vi "HOST.vi"() -> ()   [LabVIEW 2018]
uses:
  <vilib>/userdefined/High Color/nirio_resource_hc.ctl
  <instrlib>/niDCPower/nidcpower.llb/niDCPower Measurement Type.ctl
  <vilib>/FPGAPlugInAG/PXI-7953R/niLvFpga_Open_PXI-7953R.vi
  <vilib>/rvi/interface/common/dynamic/niFpgaDynamicAddResources.vi
  <vilib>/FPGAPlugInAG/Dynamic/niLvFpga_Reset_Dynamic.vi
  <vilib>/FPGAPlugInAG/Dynamic/niLvFpga_Run_Dynamic.vi
  <vilib>/Utility/error.llb/Error Cluster From Error Code.vi
  <vilib>/rvi/errors/niLvFpgaAdjustHostInterfaceError.vi
  <vilib>/FPGAPlugInAG/Dynamic/niLvFpga_Close_Dynamic.vi
  <vilib>/rvi/interface/nirviOpenFPGA/nirviOpenFPGA.xnode
  FPGA Bitfiles/KAI02050_FPGATarget_TARGET_lLVpfqL41SY.lvbitx
  <vilib>/rvi/interface/nirviMethod/nirviMethod.xnode
  <vilib>/rvi/interface/nirviReadWriteControl/nirviReadWriteControl.xnode
  <vilib>/rvi/interface/nirviCloseFPGA/nirviCloseFPGA.xnode
  NiFpgaLv.dll
  <vilib>/rvi/interface/Simulation/niFpgaSimulationCallBeginRW.vi
  <vilib>/FPGAPlugInAG/Dynamic/niLvFpga_ReadFifo_Dynamic.vi
  <vilib>/rvi/errors/niLvFpgaMergeErrorWithErrorCode.vi
panel:
  in  "LED":bool caption="output enabled"
  out "Eh":dbl
  out "Ev":dbl
  out "D, дБ":dbl
  in  "Uнас, мВ":dbl
  in  "Расчет":bool
  out "Nбд":u32
  out "Nчд":u32
  out "Картинка":bool
  out "PRNU, %":dbl
  out "DSNU, мВ, p-p":dbl
  in  "Частота, МГц?":u16=40
  in  "ISO":u16=1
  out "Vout, мВ":dbl
  in  "FPGA":T1="PXI1Slot6"
  out "Тнак, мс":dbl
  in  "Светлый (T)\nТемный (F)":bool
  in  "Frames":path=path "C:/VPL/LabView_PRJ/KAI02050/FRAMES"
  in  "ПРИМЕЧАНИЕ":string
  in  "SAVE":bool
  out "Элем.":u32
  out "Записали FIFO":bool
  out "R_LOW_char":dbl(graph)=0.00522832579698275
  out "VSUB_char":dbl(graph)=-7.684341850864879e-08
  out "STAB-15_char":dbl(graph)=0.00521525227136925
  out "STAB+15_char":dbl(graph)=-1.545303562529033e-05
  out "LED_char":dbl(graph)=5.756096264886238e-05
  out "OG_char":dbl(graph)=7.305007030606659e-07
  out "VDD_char":dbl(graph)=-4.908628444273266e-07
  out "ESD_char":dbl(graph)=-2.550812858562396e-06
  out "RD_char":dbl(graph)=-3.2917542324318195e-07
  out "ADC_char":dbl(graph)=-0.007202656860577676
  in  "MOVIE":bool
  out "Image":T2(plugin-control)
  in  "For FIFO (79)":i32=79
  out "Data":u8[][](array[numeric])
  in  "54592":u32=54592
  in  "FRAME!":bool
  in  "17850?":u16=17850
  in  "SUB2":u16=750
  in  "SUB1":u16=550
  in  "Номер SUB":u16=3
  in  "P4B_2@":u16=1700
  in  "P4B_1@":u16=1100
  in  "P4B_2@@":u16=2600
  in  "P4B_1@@":u16=2000
  in  "P1B_2_2":u16=2000
  in  "P1B_2_1":u16=1700
  in  "P1B_1_2":u16=250
  in  "P1B_1_1":u16=50
  in  "P1B_1_2@":u16=2500
  in  "P1B_1_1@":u16=1000
  in  "P4B_2":u16=350
  in  "P4B_1":u16=150
  in  "P3B_2":u16=245
  in  "P3B_1":u16=55
  in  "P3B_2@":u16=2500
  in  "P3B_1@":u16=1000
  in  "P2B_2@":u16=2600
  in  "P2B_1@":u16=1100
  in  "P2B_1":u16=155
  in  "P2B_2":u16=345
  in  "0":u16
  in  "CDS1_1":u8=1
  in  "CDS1_2":u8=4
  in  "CDS2_1":u8=5
  in  "CDS2_2":u8=10
  in  "ADC_1":u8=1
  in  "ADC_2":u8=6
  in  "17846?":u16=17846
  in  "789?":u16=789
  in  "17860?":u16=17860
  in  "P5_1":u8
  in  "P5_2":u8=6
  in  "P6_1":u8
  in  "P6_2":u8=6
  in  "P7_1":u8
  in  "P7_2":u8=2
  in  "P_end":u8=10
  in  "С_1265?":u16=1265
  in  "HIGH":u8=6
  in  "LOW":u8=1
  in  "Между кадрами, мс":u16
  in  "А(T)/А+В(F)":bool=TRUE
  in  "Линейки":bool
  in  "1":u8
  in  "2":u8
  out "Данные":u8
  in  "Направление бит":bool
  in  "4":refnum<k15>="PXI1Slot5_2" caption="1"
  in  "3":refnum<k15>="PXI1Slot4" caption="1"
  in  "2":refnum<k15>="PXI1Slot3" caption="1"
  in  "1":refnum<k15>="PXI1Slot2"
  in  "SIM_SEL":bool
  in  "R_LOW_selcur":dbl=0.01 caption="current limit" format="%_6p"
  in  "VSUB_selcur":dbl=0.01 caption="current limit" format="%_6p"
  in  "STAB-15_selcur":dbl=0.07 caption="current limit" format="%_6p"
  in  "STAB+15_selcur":dbl=0.10000000000000003 caption="current limit" format="%_6p"
  in  "LED_selcur":dbl=0.09 caption="current limit" format="%_6p"
  in  "OG_selcur":dbl=0.01 caption="current limit" format="%_6p"
  in  "VDD_selcur":dbl=0.04 caption="current limit" format="%_6p"
  in  "ESD_selcur":dbl=0.01 caption="current limit" format="%_6p"
  in  "RD_selcur":dbl=0.009999999999999997 caption="current limit" format="%_6p"
  in  "ADC_selcur":dbl=0.17 caption="current limit" format="%_6p"
  out "R_LOW":u16
  out "VSUB":u16
  out "STAB-15":u16
  out "STAB+15":u16
  out "LED":u16
  out "OG":u16
  out "VDD":u16
  out "ESD":u16
  out "RD":u16
  out "ADC":u16
  out "R_LOW":bool
  out "VSUB":bool
  out "STAB-15":bool
  out "STAB+15":bool
  out "LED":bool
  out "OG":bool
  out "VDD":bool
  out "ESD":bool
  out "RD":bool
  out "ADC":bool
  in  "Прошить АЦП":bool
  out "АЦП прошит!":bool
  in  "Какой канал?":enum16{"GREEN", "RED", "BLUE"}(ring)=enum."BLUE"
  in  "Усиление (до 6)_RED":u8=1
  in  "Усиление (до 6)_BLUE":u8=1
  in  "Усиление (до 6)_GREEN":u8=1
  in  "Смещение, до 300_BLUE":dbl
  in  "+/- BLUE":enum16{"-", "+"}(ring)=enum."+"
  in  "Смещение, до 300_RED":dbl
  in  "+/- RED":enum16{"-", "+"}(ring)=enum."+"
  in  "Смещение, до 300_GREEN":dbl
  in  "+/- GREEN":enum16{"-", "+"}(ring)=enum."+"
  in  "2/4 V":enum16{"2V", "4V"}(ring)
  in  "3CH/1CH":enum16{"3CH", "1CH"}(ring)=enum."1CH"
  out "Configuration":bool[](array[boolean])
  out "R_LOW_cur":dbl caption="measurement" format="%_6g"
  in  "R_LOW_curlim":dbl=0.015 caption="current limit" format="%_6p"
  in  "R_LOW, V":dbl=-2.0 caption="voltage level" format="%_6p"
  out "VSUB_cur":dbl caption="measurement" format="%_6g"
  in  "VSUB_curlim":dbl=0.015 caption="current limit" format="%_6p"
  in  "VSUB, V":dbl=8.0 caption="voltage level" format="%_6p"
  in  "ADC, V":dbl=6.0 caption="voltage level" format="%_6p"
  in  "VDD, V":dbl=14.900000000000004 caption="voltage level" format="%_6p"
  in  "OG, V":dbl=-2.0 caption="voltage level" format="%_6p"
  in  "STAB+15, V":dbl=15.0 caption="voltage level" format="%_6p"
  in  "ADC_curlim":dbl=0.2 caption="current limit" format="%_6p"
  in  "RD_curlim":dbl=0.045000000000000005 caption="current limit" format="%_6p"
  in  "VDD_curlim":dbl=0.1 caption="current limit" format="%_6p"
  in  "OG_curlim":dbl=0.015 caption="current limit" format="%_6p"
  in  "LED_curlim":dbl=0.1 caption="current limit" format="%_6p"
  in  "STAB+15_curlim":dbl=0.6 caption="current limit" format="%_6p"
  out "ADC_cur":dbl caption="measurement" format="%_6g"
  out "RD_cur":dbl caption="measurement" format="%_6g"
  out "VDD_cur":dbl caption="measurement" format="%_6g"
  out "OG_cur":dbl caption="measurement" format="%_6g"
  out "LED_cur":dbl caption="measurement" format="%_6g"
  out "STAB+15_cur":dbl caption="measurement" format="%_6g"
  in  "RD, V":dbl=12.0 caption="voltage level" format="%_6p"
  in  "LED, V":dbl caption="voltage level" format="%_6p"
  in  "ESD_curlim":dbl=0.015 caption="current limit" format="%_6p"
  out "ESD_cur":dbl caption="measurement" format="%_6g"
  in  "ESD, V":dbl=-9.0 caption="voltage level" format="%_6p"
  in  "STAB-15, V":dbl=-15.0 caption="voltage level" format="%_6p"
  in  "STAB-15_curlim":dbl=0.1 caption="current limit" format="%_6p"
  out "STAB-15_cur":dbl caption="measurement" format="%_6g"
  in  "Питание":bool
  in  "Стоп":bool
  out "Температура":string="0"
  in  "LOGS":path=path "C:/VPL/LabView_PRJ/KAI02050/LOGS"
  out "Номер образца":string="0"
  out "Analis":u16[][](array[numeric])
  # "ДЛЯ ТЗЧ ОПТИМАЛКА - 6 5 10 6"
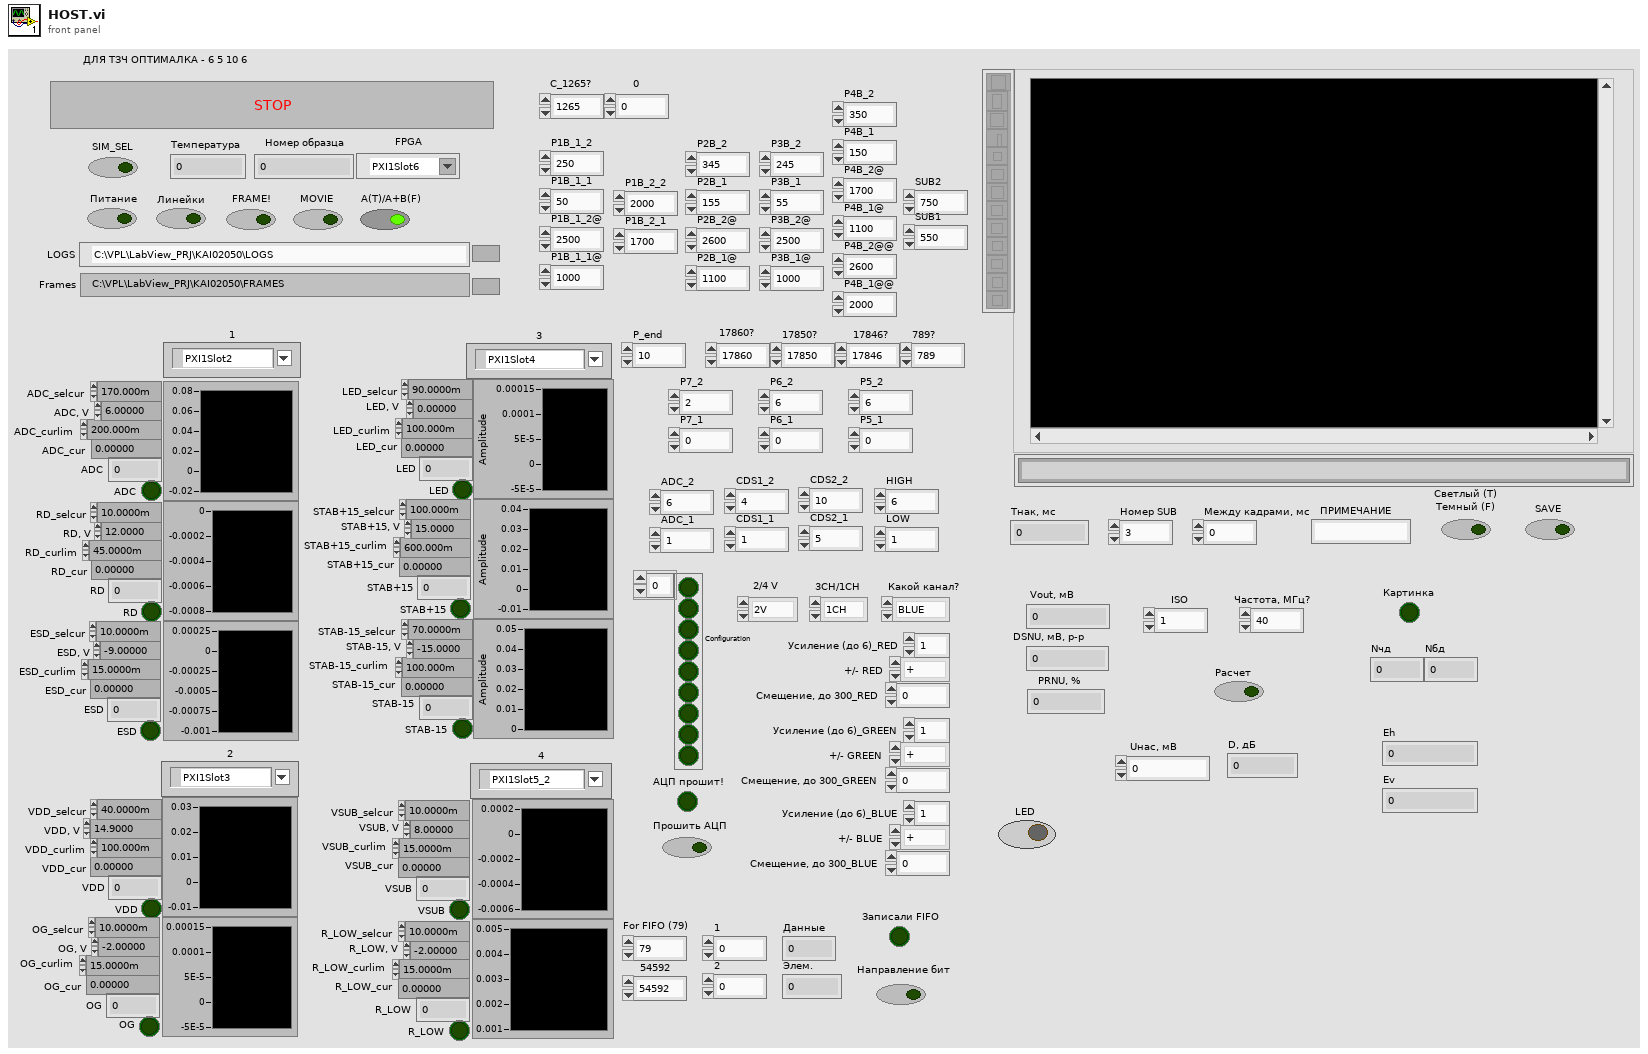
[diagram p1: front panel]
types:
  T1 = typedef "nirio_resource_hc.ctl" = tag
  T2 = typedef "IMAQ Image.ctl" = refnum<image>
  T3 = typedef "Image Type" = u32
  T4 = enum16{"open", "replace", "create", "open or create", "replace or create", "replace or create with confirmation"}
  T5 = enum16{"Configuration", "MUX", "RED PGA", "GREEN PGA", "BLUE PGA", "RED OFF", "GREEN OFF", "BLUE OFF"}
  T6 = typedef "niDCPower Measurement Type.ctl" = i32
  T7 = cluster{"Global Rectangle":i32[], "Contours":cluster{"Contour Type":u32, "ROI Type":u32, "Points":i32[]}[]}
  T8 = cluster{"Contour Type":u32, "ROI Type":u32, "Points":i32[]}[]
  T9 = cluster{"Contour Type":u32, "ROI Type":u32, "Points":i32[]}
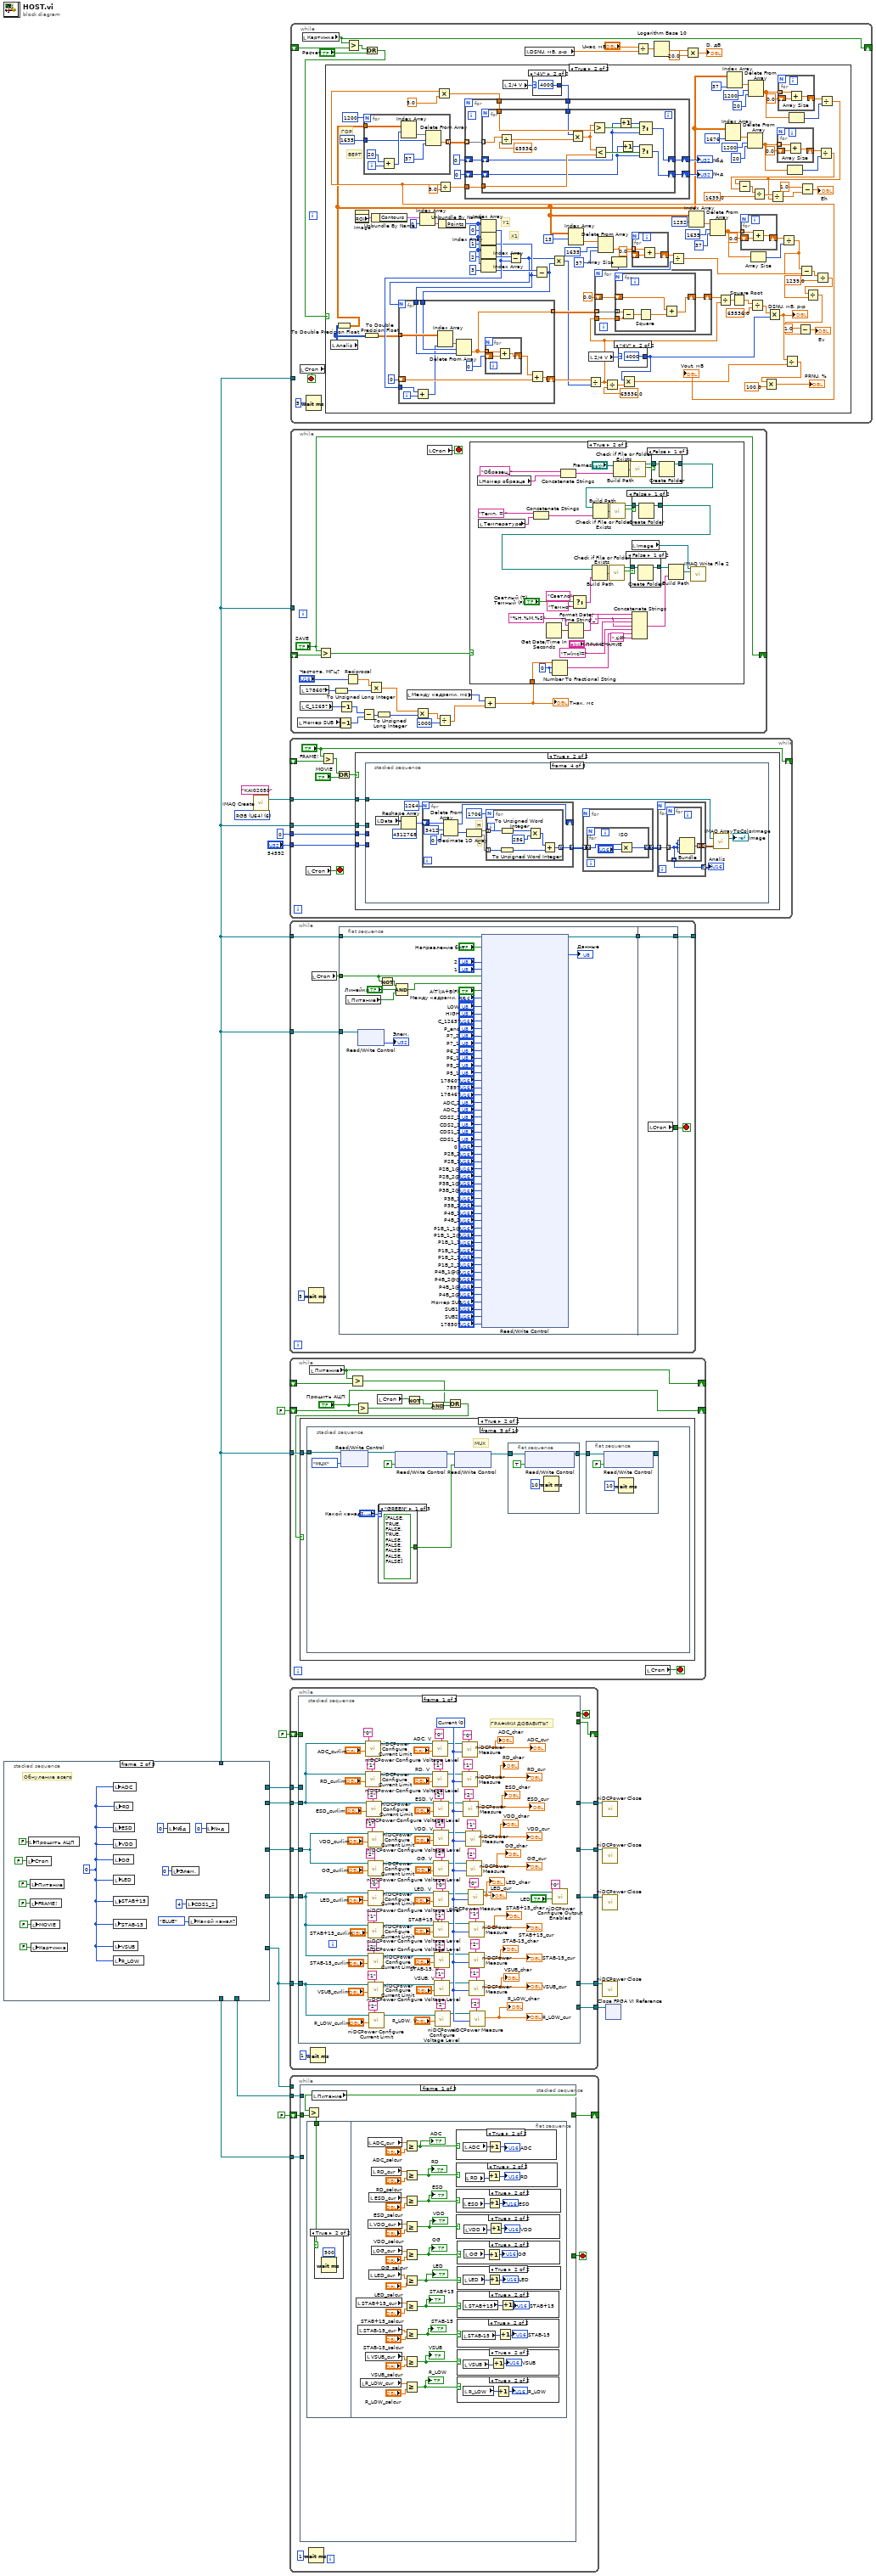
[diagram p0: block diagram]
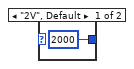
[diagram p3: hidden frame]
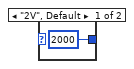
[diagram p4: hidden frame]
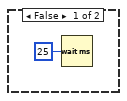
[diagram p5: hidden frame]
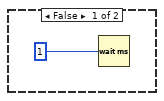
[diagram p9: hidden frame]
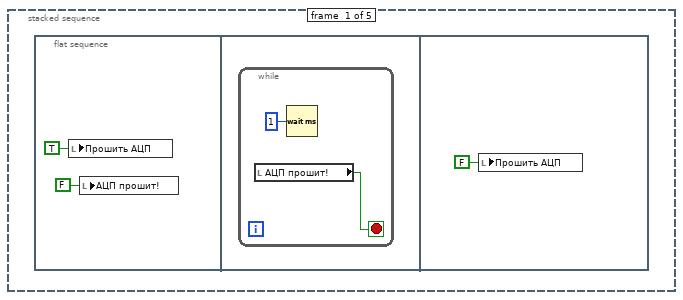
[diagram p10: hidden frame]
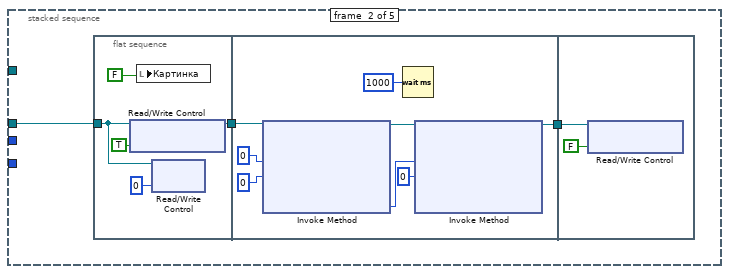
[diagram p11: hidden frame]
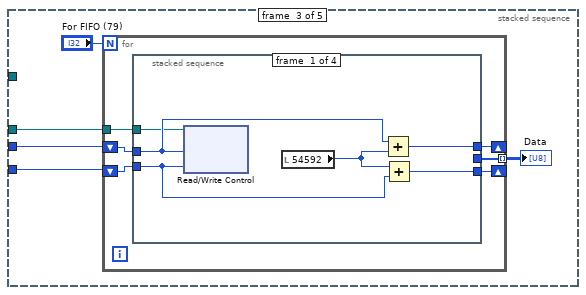
[diagram p12: hidden frame]
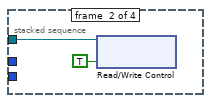
[diagram p13: hidden frame]
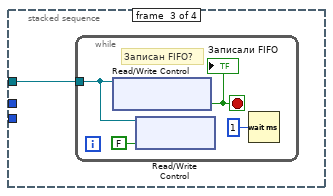
[diagram p14: hidden frame]
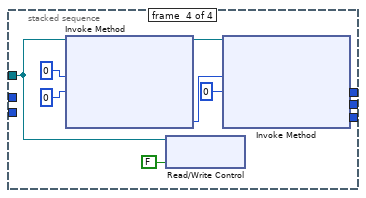
[diagram p15: hidden frame]
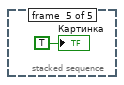
[diagram p16: hidden frame]
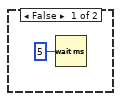
[diagram p17: hidden frame]
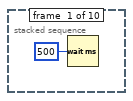
[diagram p18: hidden frame]
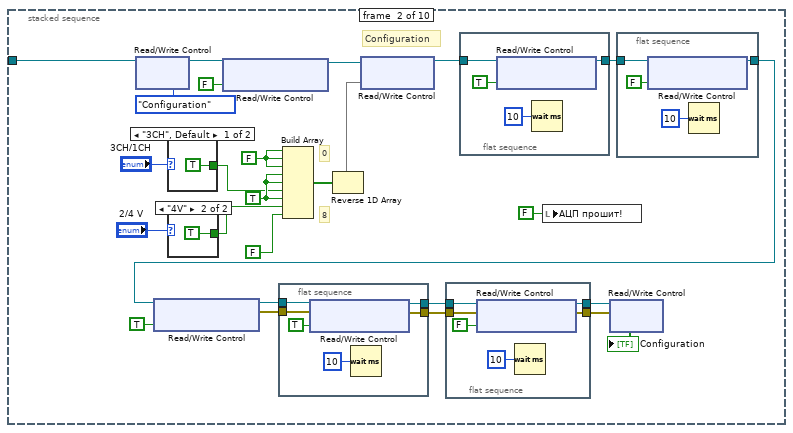
[diagram p19: hidden frame]
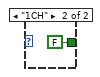
[diagram p20: hidden frame]
diagram:
  w3 = T3 6 items=["Grayscale (U8)", "Grayscale (I16)", "Grayscale (SGL)", "Complex (CSG)", "RGB (U32)", "HSL (U32)", "RGB (U64)"] ("Image Type")
  n1 = stacked-sequence {
    tunnel: [_ _ _ w83 _] -> w18
    tunnel: [_ _ _ _ w99] -> w19
    tunnel: [_ _ _ _ w98] -> w21
    tunnel: [_ _ _ _ w97] -> w20
    tunnel: [_ _ _ w83 _] -> w4
    tunnel: [_ _ _ w83 _] -> w9
    tunnel: [_ _ w49 _ _] -> w10
    tunnel: [_ _ _ _ w93] -> w11
    frame #0 {
      n2 = call "Begin.vi"() -> ("Температура 2"=→"Температура":string, "Номер образца 2"=→"Номер образца":string)  [unwired: 10 in]
    }
    frame #1 {
      w32 = u16 0 ("ADC")
      # "Обнуление всего"
      n3 = local write "Стоп"(FALSE ("Стоп")) -> ()
      n4 = local write "Прошить АЦП"(FALSE ("Прошить АЦП")) -> ()
      n5 = local write "Питание"(FALSE ("Питание")) -> ()
      n6 = local write "FRAME!"(FALSE ("FRAME!")) -> ()
      n7 = local write "MOVIE"(FALSE ("MOVIE")) -> ()
      n8 = local write "Картинка"(FALSE ("Картинка")) -> ()
      n9 = local write "ADC"(w32) -> ()
      n10 = local write "STAB-15"(w32) -> ()
      n11 = local write "VSUB"(w32) -> ()
      n12 = local write "ESD"(w32) -> ()
      n13 = local write "VDD"(w32) -> ()
      n14 = local write "OG"(w32) -> ()
      n15 = local write "LED"(w32) -> ()
      n16 = local write "STAB+15"(w32) -> ()
      n17 = local write "R_LOW"(w32) -> ()
      n18 = local write "RD"(w32) -> ()
      n19 = local write "Nбд"(0 ("Nбд")) -> ()
      n20 = local write "Элем."(u32 0 ("Элем.")) -> ()
      n21 = local write "CDS1_2"(u8 4 ("CDS1_2")) -> ()
      n22 = local write "Какой канал?"(enum16{"GREEN", "RED", "BLUE"}."BLUE" ("Какой канал?")) -> ()
      n23 = local write "Nчд"(0 ("Nчд")) -> ()
    }
    frame #2 {
      w37 = "\t"
      n24 = local read "Номер образца"() -> (w71:string)
      n25 = Build Path(base path="LOGS", name or relative path=w71) -> (appended path=w68:path)
      n26 = Get Date/Time In Seconds() -> (seconds since 1Jan1904=w65:timestamp)
      n27 = call <vilib>:"Check if File or Folder Exists.vi"("path"=w68) -> ("file or folder exists?"=w69:bool, "dup path"=w70:path)  [unwired: 8 in, 1 out]
      n28 = local read "Температура"() -> (w44:string)
      n29 = Format Date/Time String(time format string (%c)="%d %H.%M.%S", seconds (now)=w65) -> (date/time string=w63:string)  [unwired: 1 in]
      n30 = case shown="False" w69 {
        tunnel: w70 -> [w80 w81]
        tunnel: [w79 w81] -> w45
        frame False {
          n31 = Create Folder(path (use dialog)=w80) -> (created path=w79:path)  [unwired: 2 in, 2 out]
        }
        frame True {
        }
      }
      n32 = Concatenate Strings(w63, ".xls" ("string")) -> (w62:string)
      n33 = Build Path(base path=w45, name or relative path=w44) -> (appended path=w48:path)
      n34 = call <vilib>:"Check if File or Folder Exists.vi"("path"=w48) -> ("file or folder exists?"=w47:bool, "dup path"=w46:path)  [unwired: 8 in, 1 out]
      n35 = case shown="False" w47 {
        tunnel: w46 -> [w73 w74]
        tunnel: [w72 w74] -> w43
        frame False {
          n36 = Create Folder(path (use dialog)=w73) -> (created path=w72:path)  [unwired: 2 in, 2 out]
        }
        frame True {
        }
      }
      n37 = Build Path(base path=w43, name or relative path=w62) -> (appended path=w64:path)
      n38 = Open/Create/Replace File(file path (use dialog)=w64, operation (0:open)=T4."open or create", access (0:read/write)=enum16{"read/write", "read-only", "write-only"}."read/write") -> (refnum out=w66:refnum<file>)  [unwired: 3 in, 2 out]
      n39 = case shown="True" TRUE {
        tunnel: w66 -> [w75 w78]
        tunnel: [w75 w76] -> w61
        frame False {
        }
        frame True {
          n40 = Set File Position(refnum=w78, from (0:start)=enum16{"start", "end", "current"}."end") -> (refnum out=w76:refnum<file>)  [unwired: 2 in, 1 out]
        }
      }
      n41 = Format Into String(initial string=w61, "Time" ("input 1"), w37, "ADC_cur", w37, "RD_cur", w37, "ESD_cur", w37, "VDD_cur", w37, "OG_cur", w37, "LED_cur", w37, "STAB+15_cur", w37, "STAB-15_cur", w37, "VSUB_cur", w37, "R_LOW_cur", w37, "\r\n") -> (resulting string=w49:refnum<file>)  [unwired: 2 in, 1 out]
    }
    frame #3 {
      n42 = xnode "Open FPGA VI Reference"("resource name"="FPGA") -> ("FPGA VI Reference Out"=w84:refnum<k20>, "error out"=w86:errorcluster)  [unwired: 1 in]
      n43 = xnode "Invoke Method"("FPGA VI Reference In"=w84, "error in"=w86) -> ("FPGA VI Reference Out"=w87:refnum<k20>, "error out"=w85:errorcluster)
      n44 = xnode "Invoke Method"("FPGA VI Reference In"=w87, "error in"=w85) -> ("FPGA VI Reference Out"=w83:refnum<k20>)  [unwired: 1 in, 1 out]
    }
    frame #4 {
      n45 = call <instrlib>:"niDCPower Initialize.vi"("resource name"="3") -> ("error out"=w105:errorcluster, "instrument handle out"=w102:refnum<k15>)  [unwired: 3 in, 6 out]
      n46 = call <instrlib>:"niDCPower Initialize.vi"("resource name"="2") -> ("error out"=w103:errorcluster, "instrument handle out"=w100:refnum<k15>)  [unwired: 3 in, 6 out]
      n47 = call <instrlib>:"niDCPower Initialize.vi"("resource name"="4") -> ("error out"=w95:errorcluster, "instrument handle out"=w96:refnum<k15>)  [unwired: 3 in, 6 out]
      n48 = call <instrlib>:"niDCPower Initialize.vi"("resource name"="1") -> ("error out"=w104:errorcluster, "instrument handle out"=w101:refnum<k15>)  [unwired: 3 in, 6 out]
      n49 = call <instrlib>:"niDCPower Configure Voltage Level.vi"("error in (no error)"=w105, "voltage level"=0.0, "channel name"="0,1,2", "instrument handle"=w102) -> ("instrument handle out"=w99:refnum<k15>)  [unwired: 6 in, 1 out]
      n50 = call <instrlib>:"niDCPower Configure Voltage Level.vi"("error in (no error)"=w103, "voltage level"=0.0, "channel name"="0,1,2", "instrument handle"=w100) -> ("instrument handle out"=w97:refnum<k15>)  [unwired: 6 in, 1 out]
      n51 = call <instrlib>:"niDCPower Configure Voltage Level.vi"("error in (no error)"=w95, "voltage level"=0.0, "channel name"="0,1,2", "instrument handle"=w96) -> ("instrument handle out"=w93:refnum<k15>)  [unwired: 6 in, 1 out]
      n52 = call <instrlib>:"niDCPower Configure Voltage Level.vi"("error in (no error)"=w104, "voltage level"=0.0, "channel name"="0,1,2", "instrument handle"=w101) -> ("instrument handle out"=w98:refnum<k15>)  [unwired: 6 in, 1 out]
    }
  }
  n53 = call "IMAQ Create"("Image Name"="KAI02050", "Image Type"=w3) -> ("New Image"=w1:T2)  [unwired: 3 in, 1 out]
  n54 = while {
    tunnel: w4 -> [w118]
    shift-right: ["FRAME!"] -> _
    shift-left: _ -> [w120]
    tunnel: u32 0 -> [w117]
    tunnel: "54592" -> [w116]
    tunnel: w1 -> [w112]
    stop <- w121 stop-if-true
    n55 = local read "Стоп"() -> (w121:bool)
    n56 = Greater?(x="FRAME!", y=w120) -> (0:w114:bool)
    n57 = Or(x=w114, y="MOVIE") -> (x .or. y?=w115:bool)
    n58 = case shown="True" w115 {
      tunnel: w118 -> [_ w126]
      tunnel: w117 -> [_ w125]
      tunnel: w116 -> [_ w124]
      tunnel: w112 -> [_ w123]
      frame False {
        n59 = Wait (ms)(milliseconds to wait=u32 1) -> ()  [unwired: 1 out]
      }
      frame True {
        n60 = stacked-sequence {
          tunnel: w126 -> [_ w134 w154 _ _]
          tunnel: w125 -> [_ _ w153 _ _]
          tunnel: w124 -> [_ _ w152 _ _]
          tunnel: w123 -> [_ _ _ w191 _]
          frame #0 {
            n61 = flat-sequence {
              frame #0 {
                n62 = local write "Прошить АЦП"(TRUE ("Прошить АЦП")) -> ()
                n63 = local write "АЦП прошит!"(FALSE ("АЦП прошит!")) -> ()
              }
              frame #1 {
                n64 = while {
                  stop <- w130 stop-if-true
                  n65 = local read "АЦП прошит!"() -> (w130:bool)
                  n66 = Wait (ms)(milliseconds to wait=u32 1) -> ()  [unwired: 1 out]
                }
              }
              frame #2 {
                n67 = local write "Прошить АЦП"(FALSE ("Прошить АЦП")) -> ()
              }
            }
          }
          frame #1 {
            n68 = flat-sequence {
              tunnel: w134 -> [w138]
              tunnel: [w139] -> w133
              tunnel: w133 -> [w141]
              tunnel: [w140] -> w132
              tunnel: w132 -> [w148]
              frame #0 {
                n69 = xnode "Read/Write Control"("FPGA VI Reference In"=w138, "Кадр в память"=TRUE) -> ("FPGA VI Reference Out"=w139:refnum<k20>)  [unwired: 1 in, 1 out]
                n70 = local write "Картинка"(FALSE ("Картинка")) -> ()
                n71 = xnode "Read/Write Control"("FPGA VI Reference In"=w138, "Элем."=u32 0) -> ()  [unwired: 1 in, 2 out]
              }
              frame #1 {
                n72 = xnode "Invoke Method"("FPGA VI Reference In"=w141, "Number of Elements"=u32 0, "Timeout (ms)"=0) -> ("FPGA VI Reference Out"=w146:refnum<k20>, "Elements Remaining"=w145:u32)  [unwired: 1 in, 2 out]
                n73 = Wait (ms)(milliseconds to wait=u32 1000) -> ()  [unwired: 1 out]
                n74 = xnode "Invoke Method"("FPGA VI Reference In"=w146, "Number of Elements"=w145, "Timeout (ms)"=0) -> ("FPGA VI Reference Out"=w140:refnum<k20>)  [unwired: 1 in, 3 out]
              }
              frame #2 {
                n75 = xnode "Read/Write Control"("FPGA VI Reference In"=w148, "Кадр в память"=FALSE) -> ()  [unwired: 1 in, 2 out]
              }
            }
          }
          frame #2 {
            n76 = for {
              N: "For FIFO (79)" -> [_]
              shift-right: [w158] -> _
              shift-left: w153 -> [w160]
              shift-right: [w157] -> _
              shift-left: w152 -> [w159]
              tunnel: w154 -> [w156]
              tunnel: [w155] -> w151 mode=indexing
              n77 = stacked-sequence {
                tunnel: [_ _ _ w179] -> w155
                tunnel: [w166 _ _ _] -> w158
                tunnel: [w165 _ _ _] -> w157
                tunnel: w160 -> [w163 _ _ _]
                tunnel: w159 -> [w164 _ _ _]
                tunnel: w156 -> [w162 w167 w169 w174]
                frame #0 {
                  n78 = xnode "Read/Write Control"("FPGA VI Reference In"=w162, "Нач_адр"=w163, "Кон_адр"=w164) -> ()  [unwired: 1 in, 2 out]
                  n79 = local read "54592"() -> (w161:u32)
                  n80 = Add(x=w163, y=w161) -> (x+y=w166:u32)
                  n81 = Add(x=w161, y=w164) -> (x+y=w165:u32)
                }
                frame #1 {
                  n82 = xnode "Read/Write Control"("FPGA VI Reference In"=w167, "Кадр на ПК"=TRUE ("HOST")) -> ()  [unwired: 1 in, 2 out]
                }
                frame #2 {
                  n83 = while {
                    tunnel: w169 -> [w170]
                    stop <- w173 stop-if-true
                    # "Записан FIFO?"
                    n84 = xnode "Read/Write Control"("FPGA VI Reference In"=w170) -> ("Записали FIFO"=w173:bool)  [unwired: 1 in, 2 out]
                    "Записали FIFO" <- w173
                    n85 = xnode "Read/Write Control"("FPGA VI Reference In"=w170, "Кадр на ПК"=FALSE ("HOST")) -> ()  [unwired: 1 in, 2 out]
                    n86 = Wait (ms)(milliseconds to wait=u32 1) -> ()  [unwired: 1 out]
                  }
                }
                frame #3 {
                  n87 = xnode "Invoke Method"("FPGA VI Reference In"=w174, "Number of Elements"=u32 0, "Timeout (ms)"=0) -> ("FPGA VI Reference Out"=w180:refnum<k20>, "Elements Remaining"=w181:u32)  [unwired: 1 in, 2 out]
                  n88 = xnode "Read/Write Control"("FPGA VI Reference In"=w174, "Кадр на ПК"=FALSE ("HOST")) -> ()  [unwired: 1 in, 2 out]
                  n89 = xnode "Invoke Method"("FPGA VI Reference In"=w180, "Number of Elements"=w181, "Timeout (ms)"=0) -> ("Data"=w179:u8[])  [unwired: 1 in, 3 out]
                }
              }
            }
            "Data" <- w151
          }
          frame #3 {
            n90 = local read "Data"() -> (w190:u8[][])
            n91 = Reshape Array(w190, 4312768 ("dimension size")) -> (w187:u8[])
            n92 = for {
              N: 1264 -> [_]
              shift-right: [w206] -> _
              shift-left: w187 -> [w210]
              tunnel: [w202] -> w184 mode=indexing
              # "L"
              # "H"
              n93 = Delete From Array(array=w210, length=3412, index=0) -> (deleted portion=w207:u8[], array with subset deleted=w206:u8[])
              n94 = Decimate 1D Array(w207) -> (w205:u8[], w204:u8[])
              n95 = for {
                N: 1706 -> [_]
                tunnel: w205 -> [w216] mode=indexing
                tunnel: w204 -> [w217] mode=indexing
                tunnel: [w215] -> w202 mode=indexing
                n96 = To Unsigned Word Integer(number=w217) -> (unsigned 16bit integer=w211:u16)
                n97 = To Unsigned Word Integer(number=w216) -> (unsigned 16bit integer=w213:u16)
                n98 = Multiply(x=w213, y=u16 256) -> (x*y=w212:u16)
                n99 = Add(x=w212, y=w211) -> (x+y=w215:u16)
              }
            }
            n100 = for {
              tunnel: w184 -> [w193] mode=indexing
              tunnel: [w192] -> w183 mode=indexing
              n101 = for {
                tunnel: w193 -> [w196] mode=indexing
                tunnel: [w195] -> w192 mode=indexing
                n102 = Multiply(x="ISO", y=w196) -> (x*y=w195:u16)
              }
            }
            n103 = for {
              tunnel: [w199] -> w188 mode=indexing
              tunnel: w183 -> [w198] mode=indexing
              tunnel: [w197] -> w185 mode=indexing
              n104 = for {
                tunnel: w198 -> [w200] mode=indexing
                tunnel: [w201] -> w199 mode=indexing
                tunnel: [w200] -> w197 mode=indexing
                n105 = Bundle(w200, w200, w200, w200) -> (w201:cluster{u16, u16, u16, u16})  [unwired: 1 in]
              }
            }
            "Analis" <- w185
            n106 = call "IMAQ ArrayToColorImage"("Image"=w191, "Image Pixels (U64)"=w188) -> ("Image Out"=→"Image":T2)  [unwired: 3 in, 1 out]
          }
          frame #4 {
            "Картинка" <- TRUE
          }
        }
      }
    }
  }
  n107 = while {
    tunnel: w4 -> [w224]
    tunnel: [w223] -> _
    tunnel: w4 -> [w219]
    stop <- w220 stop-if-true
    n108 = Wait (ms)(milliseconds to wait=u32 5) -> ()  [unwired: 1 out]
    n109 = local read "Стоп"() -> (w222:bool)
    n110 = flat-sequence {
      tunnel: w224 -> [w282]
      tunnel: w222 -> [w229]
      tunnel: [w233] -> w221
      tunnel: w219 -> [w227]
      tunnel: [w286] -> w223
      tunnel: w221 -> [w286]
      tunnel: [w285] -> w220
      frame #0 {
        n111 = local read "Питание"() -> (w231:bool)
        n112 = xnode "Read/Write Control"("FPGA VI Reference In"=w227) -> ("Элем."=→"Элем.":u32)  [unwired: 1 in, 2 out]
        n113 = Not(x=w229) -> (.not. x?=w230:bool)
        n114 = Compound Arithmetic op=AND(w230, "Линейки", w231) -> (w228:bool)
        n115 = xnode "Read/Write Control"("FPGA VI Reference In"=w282, "Направление бит"="Направление бит", "2"="2", "1"="1", "Остановка основного цикла"=w229, "Линейки"=w228, "А(T)/А+В(F)"="А(T)/А+В(F)", "Между кадрами"="Между кадрами, мс", "LOW"="LOW", "HIGH"="HIGH", "С_1265?"="С_1265?", "P_end"="P_end", "P7_2"="P7_2", "P7_1"="P7_1", "P6_2"="P6_2", "P6_1"="P6_1", "P5_2"="P5_2", "P5_1"="P5_1", "17860?"="17860?", "789?"="789?", "17846?"="17846?", "ADC_2"="ADC_2", "ADC_1"="ADC_1", "CDS2_2"="CDS2_2", "CDS2_1"="CDS2_1", "CDS1_2"="CDS1_2", "CDS1_1"="CDS1_1", "0"="0", "P2B_2"="P2B_2", "P2B_1"="P2B_1", "P2B_1@"="P2B_1@", "P2B_2@"="P2B_2@", "P3B_1@"="P3B_1@", "P3B_2@"="P3B_2@", "P3B_1"="P3B_1", "P3B_2"="P3B_2", "P4B_1"="P4B_1", "P4B_2"="P4B_2", "P1B_1_1@"="P1B_1_1@", "P1B_1_2@"="P1B_1_2@", "P1B_1_1"="P1B_1_1", "P1B_1_2"="P1B_1_2", "P1B_2_1"="P1B_2_1", "P1B_2_2"="P1B_2_2", "P4B_1@@"="P4B_1@@", "P4B_2@@"="P4B_2@@", "P4B_1@"="P4B_1@", "P4B_2@"="P4B_2@", "Номер SUB"="Номер SUB", "SUB1"="SUB1", "SUB2"="SUB2", "17850?"="17850?") -> ("FPGA VI Reference Out"=w233:refnum<k20>, "Данные"=→"Данные":u8)  [unwired: 1 in, 1 out]
      }
      frame #1 {
        n116 = local read "Стоп"() -> (w285:bool)
      }
    }
  }
  n117 = while {
    tunnel: w4 -> [w297]
    shift-right: ["Прошить АЦП"] -> _
    shift-left: FALSE -> [w296]
    shift-right: [w291] -> _
    shift-left: _ -> [w292]
    stop <- w298 stop-if-true
    n118 = local read "Питание"() -> (w291:bool)
    n119 = Greater?(x=w291, y=w292) -> (0:w290:bool)
    n120 = Greater?(x="Прошить АЦП", y=w296) -> (0:w294:bool)
    n121 = local read "Стоп"() -> (w288:bool)
    n122 = Not(x=w288) -> (.not. x?=w287:bool)
    n123 = And(x=w287, y=w294) -> (x .and. y?=w293:bool)
    n124 = Or(x=w290, y=w293) -> (x .or. y?=w289:bool)
    n125 = case shown="True" w289 {
      tunnel: w297 -> [_ w300]
      frame False {
        n126 = Wait (ms)(milliseconds to wait=u32 5) -> ()  [unwired: 1 out]
      }
      frame True {
        n127 = stacked-sequence {
          tunnel: w300 -> [_ w327 w367 w381 w410 w454 w464 w489 w522 _]
          frame #0 {
            n128 = Wait (ms)(milliseconds to wait=u32 500) -> ()  [unwired: 1 out]
          }
          frame #1 {
            w323 = TRUE ("element")
            w324 = FALSE
            # "8"
            # "0"
            # "Configuration"
            n129 = xnode "Read/Write Control"("FPGA VI Reference In"=w327, "Enum"=T5."Configuration") -> ("FPGA VI Reference Out"=w314:refnum<k20>)  [unwired: 1 in, 1 out]
            n130 = xnode "Read/Write Control"("FPGA VI Reference In"=w304, "Read(T)/Write(F)"=TRUE) -> ("FPGA VI Reference Out"=w310:refnum<k20>, "error out"=w309:errorcluster)  [unwired: 1 in]
            n131 = case shown="\"3CH\", Default" "3CH/1CH" {
              tunnel: [TRUE FALSE] -> w322
              frame "3CH", Default {
              }
              frame "1CH" {
              }
            }
            n132 = case shown="\"4V\"" "2/4 V" {
              tunnel: [FALSE TRUE] -> w320
              frame "2V", Default {
              }
              frame "4V" {
              }
            }
            n133 = xnode "Read/Write Control"("FPGA VI Reference In"=w314, "Read(T)/Write(F)"=FALSE) -> ("FPGA VI Reference Out"=w312:refnum<k20>)  [unwired: 1 in, 1 out]
            n134 = flat-sequence {
              tunnel: w310 -> [w339]
              tunnel: w309 -> [w338]
              tunnel: [w337] -> w308
              tunnel: [w336] -> w307
              frame #0 {
                n135 = xnode "Read/Write Control"("FPGA VI Reference In"=w339, "error in"=w338, "Конфигурация"=TRUE) -> ("FPGA VI Reference Out"=w337:refnum<k20>, "error out"=w336:errorcluster)
                n136 = Wait (ms)(milliseconds to wait=u32 10) -> ()  [unwired: 1 out]
              }
            }
            n137 = Build Array(w324, w324, w324, w323, w323, w322, w323, w320, FALSE) -> (w325:bool[])
            n138 = Reverse 1D Array(array=w325) -> (reversed array=w317:bool[])
            n139 = xnode "Read/Write Control"("FPGA VI Reference In"=w312, "Write Data"=w317) -> ("FPGA VI Reference Out"=w316:refnum<k20>)  [unwired: 1 in, 1 out]
            n140 = flat-sequence {
              tunnel: w308 -> [w333]
              tunnel: w307 -> [w332]
              tunnel: [w330] -> w306
              tunnel: [w329] -> w305
              frame #0 {
                n141 = xnode "Read/Write Control"("FPGA VI Reference In"=w333, "error in"=w332, "Конфигурация"=FALSE) -> ("FPGA VI Reference Out"=w330:refnum<k20>, "error out"=w329:errorcluster)
                n142 = Wait (ms)(milliseconds to wait=u32 10) -> ()  [unwired: 1 out]
              }
            }
            n143 = flat-sequence {
              tunnel: w316 -> [w347]
              tunnel: [w345] -> w315
              frame #0 {
                n144 = xnode "Read/Write Control"("FPGA VI Reference In"=w347, "Конфигурация"=TRUE) -> ("FPGA VI Reference Out"=w345:refnum<k20>)  [unwired: 1 in, 1 out]
                n145 = Wait (ms)(milliseconds to wait=u32 10) -> ()  [unwired: 1 out]
              }
            }
            n146 = local write "АЦП прошит!"(FALSE ("АЦП прошит!")) -> ()
            n147 = xnode "Read/Write Control"("FPGA VI Reference In"=w306, "error in"=w305) -> ("READ"=→"Configuration":bool[])  [unwired: 2 out]
            n148 = flat-sequence {
              tunnel: w315 -> [w343]
              tunnel: [w341] -> w304
              frame #0 {
                n149 = xnode "Read/Write Control"("FPGA VI Reference In"=w343, "Конфигурация"=FALSE) -> ("FPGA VI Reference Out"=w341:refnum<k20>)  [unwired: 1 in, 1 out]
                n150 = Wait (ms)(milliseconds to wait=u32 10) -> ()  [unwired: 1 out]
              }
            }
          }
          frame #2 {
            # "GREEN_OFFSET"
            n151 = case shown="\"-\", Default" "+/- GREEN" {
              tunnel: [TRUE FALSE] -> w354
              frame "-", Default {
              }
              frame "+" {
              }
            }
            n152 = Quotient & Remainder(x="Смещение, до 300_GREEN", y=1.171875) -> (floor(x/y)=w359:dbl)  [unwired: 1 out]
            n153 = xnode "Read/Write Control"("FPGA VI Reference In"=w367, "Enum"=T5."GREEN OFF" ("OFFSET")) -> ("FPGA VI Reference Out"=w366:refnum<k20>, "error out"=w365:errorcluster)  [unwired: 1 in]
            n154 = Subtract(x=w359, y=1.0) -> (x-y=w356:dbl)
            n155 = To Unsigned Byte Integer(number=w356) -> (unsigned 8bit integer=w355:u8)
            n156 = xnode "Read/Write Control"("FPGA VI Reference In"=w366, "error in"=w365, "Read(T)/Write(F)"=FALSE) -> ("FPGA VI Reference Out"=w364:refnum<k20>)  [unwired: 1 out]
            n157 = Number To Boolean Array(number=w355) -> (Boolean array=w353:bool[])
            n158 = Reverse 1D Array(array=w353) -> (reversed array=w352:bool[])
            n159 = Build Array (concatenate)(w354, w352) -> (w357:bool[])
            n160 = xnode "Read/Write Control"("FPGA VI Reference In"=w364, "Write Data"=w357) -> ("FPGA VI Reference Out"=w369:refnum<k20>)  [unwired: 1 in, 1 out]
            n161 = flat-sequence {
              tunnel: w369 -> [w380]
              tunnel: [w378] -> w368
              frame #0 {
                n162 = xnode "Read/Write Control"("FPGA VI Reference In"=w380, "Конфигурация"=TRUE) -> ("FPGA VI Reference Out"=w378:refnum<k20>)  [unwired: 1 in, 1 out]
                n163 = Wait (ms)(milliseconds to wait=u32 10) -> ()  [unwired: 1 out]
              }
            }
            n164 = flat-sequence {
              tunnel: w368 -> [w376]
              tunnel: [w374] -> _
              frame #0 {
                n165 = xnode "Read/Write Control"("FPGA VI Reference In"=w376, "Конфигурация"=FALSE) -> ("FPGA VI Reference Out"=w374:refnum<k20>)  [unwired: 1 in, 1 out]
                n166 = Wait (ms)(milliseconds to wait=u32 10) -> ()  [unwired: 1 out]
              }
            }
          }
          frame #3 {
            # "RED_OFFSET"
            n167 = case shown="\"-\", Default" "+/- RED" {
              tunnel: [TRUE FALSE] -> w397
              frame "-", Default {
              }
              frame "+" {
              }
            }
            n168 = Quotient & Remainder(x="Смещение, до 300_RED", y=1.171875) -> (floor(x/y)=w392:dbl)  [unwired: 1 out]
            n169 = xnode "Read/Write Control"("FPGA VI Reference In"=w381, "Enum"=T5."RED OFF" ("OFFSET")) -> ("FPGA VI Reference Out"=w388:refnum<k20>, "error out"=w389:errorcluster)  [unwired: 1 in]
            n170 = Subtract(x=w392, y=1.0) -> (x-y=w395:dbl)
            n171 = To Unsigned Byte Integer(number=w395) -> (unsigned 8bit integer=w396:u8)
            n172 = xnode "Read/Write Control"("FPGA VI Reference In"=w388, "error in"=w389, "Read(T)/Write(F)"=FALSE) -> ("FPGA VI Reference Out"=w390:refnum<k20>)  [unwired: 1 out]
            n173 = Number To Boolean Array(number=w396) -> (Boolean array=w398:bool[])
            n174 = Reverse 1D Array(array=w398) -> (reversed array=w399:bool[])
            n175 = Build Array (concatenate)(w397, w399) -> (w394:bool[])
            n176 = xnode "Read/Write Control"("FPGA VI Reference In"=w390, "Write Data"=w394) -> ("FPGA VI Reference Out"=w386:refnum<k20>)  [unwired: 1 in, 1 out]
            n177 = flat-sequence {
              tunnel: w386 -> [w409]
              tunnel: [w407] -> w387
              frame #0 {
                n178 = xnode "Read/Write Control"("FPGA VI Reference In"=w409, "Конфигурация"=TRUE) -> ("FPGA VI Reference Out"=w407:refnum<k20>)  [unwired: 1 in, 1 out]
                n179 = Wait (ms)(milliseconds to wait=u32 10) -> ()  [unwired: 1 out]
              }
            }
            n180 = flat-sequence {
              tunnel: w387 -> [w405]
              tunnel: [w403] -> _
              frame #0 {
                n181 = xnode "Read/Write Control"("FPGA VI Reference In"=w405, "Конфигурация"=FALSE) -> ("FPGA VI Reference Out"=w403:refnum<k20>)  [unwired: 1 in, 1 out]
                n182 = Wait (ms)(milliseconds to wait=u32 10) -> ()  [unwired: 1 out]
              }
            }
          }
          frame #4 {
            # "BLUE_OFFSET"
            n183 = case shown="\"-\", Default" "+/- BLUE" {
              tunnel: [TRUE FALSE] -> w426
              frame "-", Default {
              }
              frame "+" {
              }
            }
            n184 = Quotient & Remainder(x="Смещение, до 300_BLUE", y=1.171875) -> (floor(x/y)=w421:dbl)  [unwired: 1 out]
            n185 = xnode "Read/Write Control"("FPGA VI Reference In"=w410, "Enum"=T5."BLUE OFF" ("OFFSET")) -> ("FPGA VI Reference Out"=w417:refnum<k20>, "error out"=w418:errorcluster)  [unwired: 1 in]
            n186 = Subtract(x=w421, y=1.0) -> (x-y=w424:dbl)
            n187 = To Unsigned Byte Integer(number=w424) -> (unsigned 8bit integer=w425:u8)
            n188 = xnode "Read/Write Control"("FPGA VI Reference In"=w417, "error in"=w418, "Read(T)/Write(F)"=FALSE) -> ("FPGA VI Reference Out"=w419:refnum<k20>)  [unwired: 1 out]
            n189 = Number To Boolean Array(number=w425) -> (Boolean array=w427:bool[])
            n190 = Reverse 1D Array(array=w427) -> (reversed array=w428:bool[])
            n191 = Build Array (concatenate)(w426, w428) -> (w423:bool[])
            n192 = xnode "Read/Write Control"("FPGA VI Reference In"=w419, "Write Data"=w423) -> ("FPGA VI Reference Out"=w415:refnum<k20>)  [unwired: 1 in, 1 out]
            n193 = flat-sequence {
              tunnel: w415 -> [w438]
              tunnel: [w436] -> w416
              frame #0 {
                n194 = xnode "Read/Write Control"("FPGA VI Reference In"=w438, "Конфигурация"=TRUE) -> ("FPGA VI Reference Out"=w436:refnum<k20>)  [unwired: 1 in, 1 out]
                n195 = Wait (ms)(milliseconds to wait=u32 10) -> ()  [unwired: 1 out]
              }
            }
            n196 = flat-sequence {
              tunnel: w416 -> [w434]
              tunnel: [w432] -> _
              frame #0 {
                n197 = xnode "Read/Write Control"("FPGA VI Reference In"=w434, "Конфигурация"=FALSE) -> ("FPGA VI Reference Out"=w432:refnum<k20>)  [unwired: 1 in, 1 out]
                n198 = Wait (ms)(milliseconds to wait=u32 10) -> ()  [unwired: 1 out]
              }
            }
          }
          frame #5 {
            w449 = FALSE
            # "GREEN PGA"
            n199 = Decrement(x="Усиление (до 6)_GREEN") -> (x-1=w441:u8)
            n200 = Multiply(x=w441, y=378) -> (x*y=w443:i32)
            n201 = Multiply(x="Усиление (до 6)_GREEN", y=5) -> (x*y=w446:i32)
            n202 = xnode "Read/Write Control"("FPGA VI Reference In"=w454, "Enum"=T5."GREEN PGA" ("PGA")) -> ("FPGA VI Reference Out"=w452:refnum<k20>)  [unwired: 1 in, 1 out]
            n203 = Divide(x=w443, y=w446) -> (x/y=w447:dbl)
            n204 = Number To Boolean Array(number=w447) -> (Boolean array=w440:bool[])
            n205 = xnode "Read/Write Control"("FPGA VI Reference In"=w452, "Read(T)/Write(F)"=FALSE) -> ("FPGA VI Reference Out"=w451:refnum<k20>)  [unwired: 1 in, 1 out]
            n206 = Build Array (concatenate)(w449, w449, w449, w440) -> (w448:bool[])
            n207 = xnode "Read/Write Control"("FPGA VI Reference In"=w451, "Write Data"=w448) -> ("FPGA VI Reference Out"=w453:refnum<k20>)  [unwired: 1 in, 1 out]
            n208 = flat-sequence {
              tunnel: [w462] -> w455
              tunnel: w453 -> [w461]
              frame #0 {
                n209 = xnode "Read/Write Control"("FPGA VI Reference In"=w461, "Конфигурация"=TRUE) -> ("FPGA VI Reference Out"=w462:refnum<k20>)  [unwired: 1 in, 1 out]
                n210 = Wait (ms)(milliseconds to wait=u32 10) -> ()  [unwired: 1 out]
              }
            }
            n211 = flat-sequence {
              tunnel: w455 -> [w459]
              tunnel: [w457] -> _
              frame #0 {
                n212 = xnode "Read/Write Control"("FPGA VI Reference In"=w459, "Конфигурация"=FALSE) -> ("FPGA VI Reference Out"=w457:refnum<k20>)  [unwired: 1 in, 1 out]
                n213 = Wait (ms)(milliseconds to wait=u32 10) -> ()  [unwired: 1 out]
              }
            }
          }
          frame #6 {
            w467 = FALSE
            # "BLUE PGA"
            n214 = Decrement(x="Усиление (до 6)_BLUE") -> (x-1=w471:u8)
            n215 = Multiply(x=w471, y=378) -> (x*y=w472:i32)
            n216 = Multiply(x="Усиление (до 6)_BLUE", y=5) -> (x*y=w474:i32)
            n217 = xnode "Read/Write Control"("FPGA VI Reference In"=w464, "Enum"=T5."BLUE PGA" ("PGA")) -> ("FPGA VI Reference Out"=w478:refnum<k20>)  [unwired: 1 in, 1 out]
            n218 = Divide(x=w472, y=w474) -> (x/y=w475:dbl)
            n219 = Number To Boolean Array(number=w475) -> (Boolean array=w470:bool[])
            n220 = xnode "Read/Write Control"("FPGA VI Reference In"=w478, "Read(T)/Write(F)"=FALSE) -> ("FPGA VI Reference Out"=w477:refnum<k20>)  [unwired: 1 in, 1 out]
            n221 = Build Array (concatenate)(w467, w467, w467, w470) -> (w476:bool[])
            n222 = xnode "Read/Write Control"("FPGA VI Reference In"=w477, "Write Data"=w476) -> ("FPGA VI Reference Out"=w479:refnum<k20>)  [unwired: 1 in, 1 out]
            n223 = flat-sequence {
              tunnel: [w487] -> w480
              tunnel: w479 -> [w486]
              frame #0 {
                n224 = xnode "Read/Write Control"("FPGA VI Reference In"=w486, "Конфигурация"=TRUE) -> ("FPGA VI Reference Out"=w487:refnum<k20>)  [unwired: 1 in, 1 out]
                n225 = Wait (ms)(milliseconds to wait=u32 10) -> ()  [unwired: 1 out]
              }
            }
            n226 = flat-sequence {
              tunnel: w480 -> [w484]
              tunnel: [w482] -> _
              frame #0 {
                n227 = xnode "Read/Write Control"("FPGA VI Reference In"=w484, "Конфигурация"=FALSE) -> ("FPGA VI Reference Out"=w482:refnum<k20>)  [unwired: 1 in, 1 out]
                n228 = Wait (ms)(milliseconds to wait=u32 10) -> ()  [unwired: 1 out]
              }
            }
          }
          frame #7 {
            w500 = FALSE
            # "RED PGA"
            n229 = Decrement(x="Усиление (до 6)_RED") -> (x-1=w492:u8)
            n230 = Multiply(x=w492, y=378) -> (x*y=w494:i32)
            n231 = Multiply(x="Усиление (до 6)_RED", y=5) -> (x*y=w497:i32)
            n232 = xnode "Read/Write Control"("FPGA VI Reference In"=w489, "Enum"=T5."RED PGA" ("PGA")) -> ("FPGA VI Reference Out"=w503:refnum<k20>)  [unwired: 1 in, 1 out]
            n233 = Divide(x=w494, y=w497) -> (x/y=w498:dbl)
            n234 = Number To Boolean Array(number=w498) -> (Boolean array=w491:bool[])
            n235 = xnode "Read/Write Control"("FPGA VI Reference In"=w503, "Read(T)/Write(F)"=FALSE) -> ("FPGA VI Reference Out"=w502:refnum<k20>)  [unwired: 1 in, 1 out]
            n236 = Build Array (concatenate)(w500, w500, w500, w491) -> (w499:bool[])
            n237 = xnode "Read/Write Control"("FPGA VI Reference In"=w502, "Write Data"=w499) -> ("FPGA VI Reference Out"=w504:refnum<k20>)  [unwired: 1 in, 1 out]
            n238 = flat-sequence {
              tunnel: [w512] -> w505
              tunnel: w504 -> [w511]
              frame #0 {
                n239 = xnode "Read/Write Control"("FPGA VI Reference In"=w511, "Конфигурация"=TRUE) -> ("FPGA VI Reference Out"=w512:refnum<k20>)  [unwired: 1 in, 1 out]
                n240 = Wait (ms)(milliseconds to wait=u32 10) -> ()  [unwired: 1 out]
              }
            }
            n241 = flat-sequence {
              tunnel: w505 -> [w509]
              tunnel: [w507] -> _
              frame #0 {
                n242 = xnode "Read/Write Control"("FPGA VI Reference In"=w509, "Конфигурация"=FALSE) -> ("FPGA VI Reference Out"=w507:refnum<k20>)  [unwired: 1 in, 1 out]
                n243 = Wait (ms)(milliseconds to wait=u32 10) -> ()  [unwired: 1 out]
              }
            }
          }
          frame #8 {
            # "MUX"
            n244 = xnode "Read/Write Control"("FPGA VI Reference In"=w522, "Enum"=T5."MUX") -> ("FPGA VI Reference Out"=w516:refnum<k20>)  [unwired: 1 in, 1 out]
            n245 = case shown="\"GREEN\"" "Какой канал?" {
              tunnel: [bool[] [FALSE, TRUE, FALSE, TRUE, FALSE, FALSE, FALSE, FALSE, FALSE] ("MUX_register") bool[] [FALSE, TRUE, TRUE, FALSE, FALSE, FALSE, FALSE, FALSE, FALSE] ("MUX_register") bool[] [FALSE, TRUE, FALSE, FALSE, TRUE, FALSE, FALSE, FALSE, FALSE] ("MUX_register")] -> w514
              frame "GREEN" {
              }
              frame "RED", Default {
              }
              frame "BLUE" {
              }
            }
            n246 = xnode "Read/Write Control"("FPGA VI Reference In"=w516, "Read(T)/Write(F)"=FALSE) -> ("FPGA VI Reference Out"=w518:refnum<k20>)  [unwired: 1 in, 1 out]
            n247 = xnode "Read/Write Control"("FPGA VI Reference In"=w518, "Write Data"=w514) -> ("FPGA VI Reference Out"=w519:refnum<k20>)  [unwired: 1 in, 1 out]
            n248 = flat-sequence {
              tunnel: [w532] -> w520
              tunnel: w519 -> [w531]
              frame #0 {
                n249 = xnode "Read/Write Control"("FPGA VI Reference In"=w531, "Конфигурация"=TRUE) -> ("FPGA VI Reference Out"=w532:refnum<k20>)  [unwired: 1 in, 1 out]
                n250 = Wait (ms)(milliseconds to wait=u32 10) -> ()  [unwired: 1 out]
              }
            }
            n251 = flat-sequence {
              tunnel: w520 -> [w529]
              tunnel: [w527] -> _
              frame #0 {
                n252 = xnode "Read/Write Control"("FPGA VI Reference In"=w529, "Конфигурация"=FALSE) -> ("FPGA VI Reference Out"=w527:refnum<k20>)  [unwired: 1 in, 1 out]
                n253 = Wait (ms)(milliseconds to wait=u32 10) -> ()  [unwired: 1 out]
              }
            }
          }
          frame #9 {
            "АЦП прошит!" <- TRUE ("АЦП прошит!")
          }
        }
      }
    }
    n254 = local read "Стоп"() -> (w298:bool)
  }
  n255 = while {
    tunnel: w21 -> [w547]
    tunnel: w20 -> [w546]
    tunnel: w19 -> [w545]
    tunnel: w11 -> [w543]
    tunnel: w18 -> [w536]
    shift-right: [w541] -> _
    shift-left: FALSE -> [w542]
    tunnel: [w540] -> w16
    tunnel: [w539] -> w14
    tunnel: [w538] -> w13
    tunnel: [w537] -> w15
    tunnel: [w535] -> w5
    stop <- w544 stop-if-true
    n256 = stacked-sequence {
      tunnel: w545 -> [w563 w641 w716]
      tunnel: w547 -> [w565 w643 w718]
      tunnel: w546 -> [w564 w642 w717]
      tunnel: [_ "Стоп" _] -> w544
      tunnel: w543 -> [w562 w640 w715]
      tunnel: w542 -> [_ w649 _]
      tunnel: [_ "Питание" _] -> w541
      tunnel: [_ _ w718] -> w540
      tunnel: [_ _ w717] -> w539
      tunnel: [_ _ w716] -> w538
      tunnel: [_ _ w715] -> w537
      tunnel: w536 -> [_ w639 _]
      tunnel: [_ w637 _] -> w535
      frame #0 {
        w576 = T6 0 items=["Current", "Voltage"] ("measurement type")
        # "ГРАФИКИ ДОБАВИТЬ?"
        n257 = call <instrlib>:"niDCPower Configure Current Limit.vi"("current limit"="ADC_curlim", "channel name"="0", "instrument handle"=w565) -> ("instrument handle out"=w617:refnum<k15>)  [unwired: 7 in, 1 out]
        n258 = call <instrlib>:"niDCPower Configure Current Limit.vi"("current limit"="RD_curlim", "channel name"="1", "instrument handle"=w565) -> ("instrument handle out"=w618:refnum<k15>)  [unwired: 7 in, 1 out]
        n259 = call <instrlib>:"niDCPower Configure Current Limit.vi"("current limit"="ESD_curlim", "channel name"="2", "instrument handle"=w565) -> ("instrument handle out"=w598:refnum<k15>)  [unwired: 7 in, 1 out]
        n260 = call <instrlib>:"niDCPower Configure Current Limit.vi"("current limit"="VDD_curlim", "channel name"="1", "instrument handle"=w564) -> ("instrument handle out"=w619:refnum<k15>)  [unwired: 7 in, 1 out]
        n261 = call <instrlib>:"niDCPower Configure Current Limit.vi"("current limit"="OG_curlim", "channel name"="2", "instrument handle"=w564) -> ("instrument handle out"=w620:refnum<k15>)  [unwired: 7 in, 1 out]
        n262 = call <instrlib>:"niDCPower Configure Current Limit.vi"("current limit"="LED_curlim", "channel name"="0", "instrument handle"=w563) -> ("instrument handle out"=w621:refnum<k15>)  [unwired: 7 in, 1 out]
        n263 = call <instrlib>:"niDCPower Configure Current Limit.vi"("current limit"="STAB+15_curlim", "channel name"="1", "instrument handle"=w563) -> ("instrument handle out"=w622:refnum<k15>)  [unwired: 7 in, 1 out]
        n264 = call <instrlib>:"niDCPower Configure Current Limit.vi"("current limit"="STAB-15_curlim", "channel name"="2", "instrument handle"=w563) -> ("instrument handle out"=w591:refnum<k15>)  [unwired: 7 in, 1 out]
        n265 = call <instrlib>:"niDCPower Configure Current Limit.vi"("current limit"="VSUB_curlim", "channel name"="1", "instrument handle"=w562) -> ("instrument handle out"=w584:refnum<k15>)  [unwired: 7 in, 1 out]
        n266 = call <instrlib>:"niDCPower Configure Current Limit.vi"("current limit"="R_LOW_curlim", "channel name"="2", "instrument handle"=w562) -> ("instrument handle out"=w587:refnum<k15>)  [unwired: 7 in, 1 out]
        n267 = call <instrlib>:"niDCPower Configure Voltage Level.vi"("voltage level"="ADC, V", "channel name"="0", "instrument handle"=w617) -> ("instrument handle out"=w575:refnum<k15>)  [unwired: 7 in, 1 out]
        n268 = call <instrlib>:"niDCPower Configure Voltage Level.vi"("voltage level"="RD, V", "channel name"="1", "instrument handle"=w618) -> ("instrument handle out"=w574:refnum<k15>)  [unwired: 7 in, 1 out]
        n269 = call <instrlib>:"niDCPower Configure Voltage Level.vi"("voltage level"="ESD, V", "channel name"="2", "instrument handle"=w598) -> ("instrument handle out"=w573:refnum<k15>)  [unwired: 7 in, 1 out]
        n270 = call <instrlib>:"niDCPower Configure Voltage Level.vi"("voltage level"="VDD, V", "channel name"="1", "instrument handle"=w619) -> ("instrument handle out"=w572:refnum<k15>)  [unwired: 7 in, 1 out]
        n271 = call <instrlib>:"niDCPower Configure Voltage Level.vi"("voltage level"="OG, V", "channel name"="2", "instrument handle"=w620) -> ("instrument handle out"=w571:refnum<k15>)  [unwired: 7 in, 1 out]
        n272 = call <instrlib>:"niDCPower Configure Voltage Level.vi"("voltage level"="LED, V", "channel name"="0", "instrument handle"=w621) -> ("instrument handle out"=w570:refnum<k15>)  [unwired: 7 in, 1 out]
        n273 = call <instrlib>:"niDCPower Configure Voltage Level.vi"("voltage level"="STAB+15, V", "channel name"="1", "instrument handle"=w622) -> ("instrument handle out"=w569:refnum<k15>)  [unwired: 7 in, 1 out]
        n274 = call <instrlib>:"niDCPower Configure Voltage Level.vi"("voltage level"="STAB-15, V", "channel name"="2", "instrument handle"=w591) -> ("instrument handle out"=w568:refnum<k15>)  [unwired: 7 in, 1 out]
        n275 = call <instrlib>:"niDCPower Configure Voltage Level.vi"("voltage level"="VSUB, V", "channel name"="1", "instrument handle"=w584) -> ("instrument handle out"=w567:refnum<k15>)  [unwired: 7 in, 1 out]
        n276 = call <instrlib>:"niDCPower Configure Voltage Level.vi"("voltage level"="R_LOW, V", "channel name"="2", "instrument handle"=w587) -> ("instrument handle out"=w566:refnum<k15>)  [unwired: 7 in, 1 out]
        n277 = call <instrlib>:"niDCPower Measure.vi"("measurement type"=w576, "channel name"="0", "instrument handle"=w575) -> ("measurement"=→"ADC_cur" →"ADC_char":dbl)  [unwired: 6 in, 2 out]
        n278 = call <instrlib>:"niDCPower Measure.vi"("measurement type"=w576, "channel name"="1", "instrument handle"=w574) -> ("measurement"=→"RD_cur" →"RD_char":dbl)  [unwired: 6 in, 2 out]
        n279 = call <instrlib>:"niDCPower Measure.vi"("measurement type"=w576, "channel name"="2", "instrument handle"=w573) -> ("measurement"=→"ESD_cur" →"ESD_char":dbl)  [unwired: 6 in, 2 out]
        n280 = call <instrlib>:"niDCPower Measure.vi"("measurement type"=w576, "channel name"="1", "instrument handle"=w572) -> ("measurement"=→"VDD_cur" →"VDD_char":dbl)  [unwired: 6 in, 2 out]
        n281 = call <instrlib>:"niDCPower Measure.vi"("measurement type"=w576, "channel name"="2", "instrument handle"=w571) -> ("measurement"=→"OG_cur" →"OG_char":dbl)  [unwired: 6 in, 2 out]
        n282 = call <instrlib>:"niDCPower Measure.vi"("measurement type"=w576, "channel name"="0", "instrument handle"=w570) -> ("measurement"=→"LED_cur" →"LED_char":dbl, "instrument handle out"=w551:refnum<k15>)  [unwired: 6 in, 1 out]
        n283 = call <instrlib>:"niDCPower Measure.vi"("measurement type"=w576, "channel name"="1", "instrument handle"=w569) -> ("measurement"=→"STAB+15_cur" →"STAB+15_char":dbl)  [unwired: 6 in, 2 out]
        n284 = call <instrlib>:"niDCPower Measure.vi"("measurement type"=w576, "channel name"="2", "instrument handle"=w568) -> ("measurement"=→"STAB-15_cur" →"STAB-15_char":dbl)  [unwired: 6 in, 2 out]
        n285 = call <instrlib>:"niDCPower Measure.vi"("measurement type"=w576, "channel name"="1", "instrument handle"=w567) -> ("measurement"=→"VSUB_cur" →"VSUB_char":dbl)  [unwired: 6 in, 2 out]
        n286 = call <instrlib>:"niDCPower Measure.vi"("measurement type"=w576, "channel name"="2", "instrument handle"=w566) -> ("measurement"=→"R_LOW_cur" →"R_LOW_char":dbl)  [unwired: 6 in, 2 out]
        n287 = call <instrlib>:"niDCPower Configure Output Enabled.vi"("output enabled"="LED", "channel name"="0", "instrument handle"=w551) -> ()  [unwired: 7 in, 2 out]
      }
      frame #1 {
        n288 = Greater?(x="Питание", y=w649) -> (0:w646:bool)
        n289 = Less?(x="Питание", y=w649) -> (x < y?=w644:bool)
        n290 = Not(x="Стоп") -> (.not. x?=w645:bool)
        n291 = And(x=w645, y=w646) -> (x .and. y?=w648:bool)
        n292 = Or(x="Стоп", y=w644) -> (x .or. y?=w647:bool)
        n293 = case shown="False" w647 {
          tunnel: w643 -> [_ w657]
          tunnel: w642 -> [_ w656]
          tunnel: w641 -> [_ w655]
          tunnel: w640 -> [_ w654]
          tunnel: w639 -> [w651 w653]
          tunnel: [w651 w652] -> w637
          frame False {
          }
          frame True {
            # "Выключение"
            n294 = stacked-sequence {
              tunnel: w657 -> [w663 _ w681]
              tunnel: w656 -> [w662 _ _]
              tunnel: w655 -> [w661 _ _]
              tunnel: w654 -> [w660 _ w680]
              tunnel: w653 -> [w658 _ w679]
              tunnel: [_ _ w679] -> w652
              frame #0 {
                n295 = call <instrlib>:"niDCPower Configure Output Enabled.vi"("output enabled"=FALSE, "channel name"="2", "instrument handle"=w660) -> ()  [unwired: 7 in, 2 out]
                n296 = xnode "Read/Write Control"("FPGA VI Reference In"=w658, "Линейки"=FALSE) -> ()  [unwired: 1 in, 2 out]
                n297 = call <instrlib>:"niDCPower Configure Output Enabled.vi"("output enabled"=FALSE, "channel name"="1", "instrument handle"=w661) -> ()  [unwired: 7 in, 2 out]
                n298 = call <instrlib>:"niDCPower Configure Output Enabled.vi"("output enabled"=FALSE, "channel name"="2", "instrument handle"=w661) -> ()  [unwired: 7 in, 2 out]
                n299 = call <instrlib>:"niDCPower Configure Output Enabled.vi"("output enabled"=FALSE, "channel name"="1", "instrument handle"=w662) -> ()  [unwired: 7 in, 2 out]
                n300 = call <instrlib>:"niDCPower Configure Output Enabled.vi"("output enabled"=FALSE, "channel name"="2", "instrument handle"=w662) -> ()  [unwired: 7 in, 2 out]
                n301 = call <instrlib>:"niDCPower Configure Output Enabled.vi"("output enabled"=FALSE, "channel name"="0", "instrument handle"=w663) -> ()  [unwired: 7 in, 2 out]
                n302 = call <instrlib>:"niDCPower Configure Output Enabled.vi"("output enabled"=FALSE, "channel name"="1", "instrument handle"=w663) -> ()  [unwired: 7 in, 2 out]
              }
              frame #1 {
                n303 = Wait (ms)(milliseconds to wait=u32 200) -> ()  [unwired: 1 out]
              }
              frame #2 {
                # "VSUB"
                # "ESD"
                n304 = call <instrlib>:"niDCPower Configure Output Enabled.vi"("output enabled"=FALSE, "channel name"="1", "instrument handle"=w680) -> ()  [unwired: 7 in, 2 out]
                n305 = call <instrlib>:"niDCPower Configure Output Enabled.vi"("output enabled"=FALSE, "channel name"="2", "instrument handle"=w681) -> ()  [unwired: 7 in, 2 out]
              }
            }
          }
        }
        n306 = case shown="True" w648 {
          tunnel: w643 -> [_ w689]
          tunnel: w642 -> [_ w688]
          tunnel: w641 -> [_ w687]
          tunnel: w640 -> [_ w686]
          frame False {
          }
          frame True {
            # "Включение"
            n307 = stacked-sequence {
              tunnel: w689 -> [w693 _ w706]
              tunnel: w688 -> [_ _ w705]
              tunnel: w687 -> [_ _ w704]
              tunnel: w686 -> [w691 _ w707]
              frame #0 {
                # "VSUB"
                # "ESD"
                n308 = call <instrlib>:"niDCPower Configure Output Enabled.vi"("output enabled"=TRUE, "channel name"="1", "instrument handle"=w691) -> ()  [unwired: 7 in, 2 out]
                n309 = call <instrlib>:"niDCPower Configure Output Enabled.vi"("output enabled"=TRUE, "channel name"="2", "instrument handle"=w693) -> ()  [unwired: 7 in, 2 out]
              }
              frame #1 {
                n310 = Wait (ms)(milliseconds to wait=u32 200) -> ()  [unwired: 1 out]
              }
              frame #2 {
                n311 = call <instrlib>:"niDCPower Configure Output Enabled.vi"("output enabled"=TRUE, "channel name"="2", "instrument handle"=w707) -> ()  [unwired: 7 in, 2 out]
                n312 = call <instrlib>:"niDCPower Configure Output Enabled.vi"("output enabled"=TRUE, "channel name"="1", "instrument handle"=w704) -> ()  [unwired: 7 in, 2 out]
                n313 = call <instrlib>:"niDCPower Configure Output Enabled.vi"("output enabled"=TRUE, "channel name"="2", "instrument handle"=w704) -> ()  [unwired: 7 in, 2 out]
                n314 = call <instrlib>:"niDCPower Configure Output Enabled.vi"("output enabled"=TRUE, "channel name"="1", "instrument handle"=w705) -> ()  [unwired: 7 in, 2 out]
                n315 = call <instrlib>:"niDCPower Configure Output Enabled.vi"("output enabled"=TRUE, "channel name"="2", "instrument handle"=w705) -> ()  [unwired: 7 in, 2 out]
                n316 = call <instrlib>:"niDCPower Configure Output Enabled.vi"("output enabled"=TRUE, "channel name"="0", "instrument handle"=w706) -> ()  [unwired: 7 in, 2 out]
                n317 = call <instrlib>:"niDCPower Configure Output Enabled.vi"("output enabled"=TRUE, "channel name"="1", "instrument handle"=w706) -> ()  [unwired: 7 in, 2 out]
              }
            }
          }
        }
      }
      frame #2 {
      }
    }
    n318 = Wait (ms)(milliseconds to wait=u32 1) -> ()  [unwired: 1 out]
  }
  n319 = while {
    tunnel: w9 -> [w719]
    shift-right: [w723] -> _
    shift-left: FALSE ("Питание") -> [w724]
    tunnel: w11 -> [_]
    tunnel: w10 -> [w721]
    stop <- w720 stop-if-true
    n320 = stacked-sequence {
      tunnel: w724 -> [w727 _ _]
      tunnel: [w726 _ _] -> w723
      tunnel: w721 -> [_ w826 _]
      tunnel: [_ _ w844] -> w720
      tunnel: w719 -> [_ _ w843]
      frame #0 {
        n321 = flat-sequence {
          tunnel: w725 -> [w728]
          frame #0 {
            n322 = case shown="True" w728 {
              frame False {
              }
              frame True {
                n323 = Wait (ms)(milliseconds to wait=u32 500) -> ()  [unwired: 1 out]
              }
            }
          }
          frame #1 {
            n324 = local read "STAB+15_cur"() -> (w746:dbl)
            n325 = local read "STAB-15_cur"() -> (w745:dbl)
            n326 = local read "R_LOW_cur"() -> (w741:dbl)
            n327 = local read "VSUB_cur"() -> (w743:dbl)
            n328 = local read "ADC_cur"() -> (w750:dbl)
            n329 = local read "VDD_cur"() -> (w753:dbl)
            n330 = local read "ESD_cur"() -> (w752:dbl)
            n331 = local read "LED_cur"() -> (w749:dbl)
            n332 = local read "OG_cur"() -> (w754:dbl)
            n333 = local read "RD_cur"() -> (w751:dbl)
            n334 = Greater Or Equal?(x=w750, y="ADC_selcur") -> (x >= y?=w739:bool)
            "ADC" <- w739
            n335 = Greater Or Equal?(x=w751, y="RD_selcur") -> (x >= y?=w738:bool)
            "RD" <- w738
            n336 = Greater Or Equal?(x=w752, y="ESD_selcur") -> (x >= y?=w737:bool)
            "ESD" <- w737
            n337 = Greater Or Equal?(x=w753, y="VDD_selcur") -> (x >= y?=w736:bool)
            "VDD" <- w736
            n338 = Greater Or Equal?(x=w754, y="OG_selcur") -> (x >= y?=w735:bool)
            "OG" <- w735
            n339 = Greater Or Equal?(x=w749, y="LED_selcur") -> (x >= y?=w734:bool)
            "LED" <- w734
            n340 = Greater Or Equal?(x=w746, y="STAB+15_selcur") -> (x >= y?=w733:bool)
            "STAB+15" <- w733
            n341 = Greater Or Equal?(x=w745, y="STAB-15_selcur") -> (x >= y?=w732:bool)
            "STAB-15" <- w732
            n342 = Greater Or Equal?(x=w743, y="VSUB_selcur") -> (x >= y?=w731:bool)
            "VSUB" <- w731
            n343 = Greater Or Equal?(x=w741, y="R_LOW_selcur") -> (x >= y?=w730:bool)
            "R_LOW" <- w730
            n344 = case shown="True" w739 {
              frame False {
              }
              frame True {
                n345 = local read "ADC"() -> (w778:u16)
                n346 = Increment(x=w778) -> (x+1=→"ADC":u16)
              }
            }
            n347 = case shown="True" w738 {
              frame False {
              }
              frame True {
                n348 = local read "RD"() -> (w776:u16)
                n349 = Increment(x=w776) -> (x+1=→"RD":u16)
              }
            }
            n350 = case shown="True" w737 {
              frame False {
              }
              frame True {
                n351 = local read "ESD"() -> (w774:u16)
                n352 = Increment(x=w774) -> (x+1=→"ESD":u16)
              }
            }
            n353 = case shown="True" w736 {
              frame False {
              }
              frame True {
                n354 = local read "VDD"() -> (w772:u16)
                n355 = Increment(x=w772) -> (x+1=→"VDD":u16)
              }
            }
            n356 = case shown="True" w735 {
              frame False {
              }
              frame True {
                n357 = local read "OG"() -> (w770:u16)
                n358 = Increment(x=w770) -> (x+1=→"OG":u16)
              }
            }
            n359 = case shown="True" w734 {
              frame False {
              }
              frame True {
                n360 = local read "LED"() -> (w768:u16)
                n361 = Increment(x=w768) -> (x+1=→"LED":u16)
              }
            }
            n362 = case shown="True" w732 {
              frame False {
              }
              frame True {
                n363 = local read "STAB-15"() -> (w764:u16)
                n364 = Increment(x=w764) -> (x+1=→"STAB-15":u16)
              }
            }
            n365 = case shown="True" w733 {
              frame False {
              }
              frame True {
                n366 = local read "STAB+15"() -> (w766:u16)
                n367 = Increment(x=w766) -> (x+1=→"STAB+15":u16)
              }
            }
            n368 = case shown="True" w731 {
              frame False {
              }
              frame True {
                n369 = local read "VSUB"() -> (w762:u16)
                n370 = Increment(x=w762) -> (x+1=→"VSUB":u16)
              }
            }
            n371 = case shown="True" w730 {
              frame False {
              }
              frame True {
                n372 = local read "R_LOW"() -> (w760:u16)
                n373 = Increment(x=w760) -> (x+1=→"R_LOW":u16)
              }
            }
          }
        }
        n374 = local read "Питание"() -> (w726:bool)
        n375 = Greater?(x=w726, y=w727) -> (0:w725:bool)
      }
      frame #1 {
        w812 = "\t"
        w824 = i16 0 ("width (-)")
        w825 = i16 3 ("width (-)")
        n376 = local read "STAB+15"() -> (w831:bool)
        n377 = local read "STAB+15_cur"() -> (w816:dbl)
        n378 = local read "STAB-15"() -> (w830:bool)
        n379 = local read "STAB-15_cur"() -> (w815:dbl)
        n380 = local read "STAB+15"() -> (w805:u16)
        n381 = local read "R_LOW"() -> (w828:bool)
        n382 = local read "R_LOW_cur"() -> (w813:dbl)
        n383 = local read "STAB-15"() -> (w804:u16)
        n384 = local read "R_LOW"() -> (w802:u16)
        n385 = local read "VSUB"() -> (w829:bool)
        n386 = local read "VSUB_cur"() -> (w814:dbl)
        n387 = local read "ADC"() -> (w837:bool)
        n388 = local read "VDD"() -> (w834:bool)
        n389 = local read "ADC_cur"() -> (w822:dbl)
        n390 = local read "ESD"() -> (w835:bool)
        n391 = local read "VDD_cur"() -> (w819:dbl)
        n392 = local read "VSUB"() -> (w803:u16)
        n393 = local read "LED"() -> (w832:bool)
        n394 = local read "ESD_cur"() -> (w820:dbl)
        n395 = local read "LED_cur"() -> (w817:dbl)
        n396 = local read "OG"() -> (w833:bool)
        n397 = local read "ADC"() -> (w811:u16)
        n398 = local read "RD"() -> (w836:bool)
        n399 = local read "OG_cur"() -> (w818:dbl)
        n400 = local read "VDD"() -> (w808:u16)
        n401 = local read "RD_cur"() -> (w821:dbl)
        n402 = local read "ESD"() -> (w809:u16)
        n403 = local read "LED"() -> (w806:u16)
        n404 = local read "OG"() -> (w807:u16)
        n405 = local read "RD"() -> (w810:u16)
        n406 = Get Date/Time In Seconds() -> (seconds since 1Jan1904=w842:timestamp)
        n407 = Format Date/Time String(time format string (%c)="%d %H:%M:%S:%3u", seconds (now)=w842) -> (date/time string=w823:string)  [unwired: 1 in]
        n408 = Compound Arithmetic op=OR(w837, w836, w835, w834, w833, w832, w831, w830, w829, w828) -> (w840:bool)
        n409 = Select(t="!!!", s=w840, f="") -> (s? t:f=w781:string)
        n410 = Number To Fractional String(number=w822, width (-)=w825, precision (6)=w825) -> (F-format string=w801:string)  [unwired: 1 in]
        n411 = Number To Fractional String(number=w821, width (-)=w825, precision (6)=w825) -> (F-format string=w800:string)  [unwired: 1 in]
        n412 = Number To Fractional String(number=w820, width (-)=w825, precision (6)=w825) -> (F-format string=w799:string)  [unwired: 1 in]
        n413 = Number To Fractional String(number=w819, width (-)=w825, precision (6)=w825) -> (F-format string=w798:string)  [unwired: 1 in]
        n414 = Number To Fractional String(number=w818, width (-)=w825, precision (6)=w825) -> (F-format string=w797:string)  [unwired: 1 in]
        n415 = Number To Fractional String(number=w817, width (-)=w825, precision (6)=w825) -> (F-format string=w796:string)  [unwired: 1 in]
        n416 = Number To Fractional String(number=w816, width (-)=w825, precision (6)=w825) -> (F-format string=w795:string)  [unwired: 1 in]
        n417 = Number To Fractional String(number=w815, width (-)=w825, precision (6)=w825) -> (F-format string=w794:string)  [unwired: 1 in]
        n418 = Number To Fractional String(number=w814, width (-)=w825, precision (6)=w825) -> (F-format string=w793:string)  [unwired: 1 in]
        n419 = Number To Fractional String(number=w813, width (-)=w825, precision (6)=w825) -> (F-format string=w792:string)  [unwired: 1 in]
        n420 = Number To Fractional String(number=w811, width (-)=w824, precision (6)=w824) -> (F-format string=w791:string)  [unwired: 1 in]
        n421 = Number To Fractional String(number=w810, width (-)=w824, precision (6)=w824) -> (F-format string=w790:string)  [unwired: 1 in]
        n422 = Number To Fractional String(number=w809, width (-)=w824, precision (6)=w824) -> (F-format string=w789:string)  [unwired: 1 in]
        n423 = Number To Fractional String(number=w808, width (-)=w824, precision (6)=w824) -> (F-format string=w788:string)  [unwired: 1 in]
        n424 = Number To Fractional String(number=w807, width (-)=w824, precision (6)=w824) -> (F-format string=w787:string)  [unwired: 1 in]
        n425 = Number To Fractional String(number=w806, width (-)=w824, precision (6)=w824) -> (F-format string=w786:string)  [unwired: 1 in]
        n426 = Number To Fractional String(number=w805, width (-)=w824, precision (6)=w824) -> (F-format string=w785:string)  [unwired: 1 in]
        n427 = Number To Fractional String(number=w804, width (-)=w824, precision (6)=w824) -> (F-format string=w784:string)  [unwired: 1 in]
        n428 = Number To Fractional String(number=w803, width (-)=w824, precision (6)=w824) -> (F-format string=w783:string)  [unwired: 1 in]
        n429 = Number To Fractional String(number=w802, width (-)=w824, precision (6)=w824) -> (F-format string=w782:string)  [unwired: 1 in]
        n430 = Concatenate Strings(w823, w812, w801, w812, w800, w812, w799, w812, w798, w812, w797, w812, w796, w812, w795, w812, w794, w812, w793, w812, w792, w812, w791, w812, w790, w812, w789, w812, w788, w812, w787, w812, w786, w812, w785, w812, w784, w812, w783, w812, w782, w812, w781, "\r\n") -> (w827:string)
        n431 = Format Into String(initial string=w826, w827) -> ()  [unwired: 2 in, 2 out]
      }
      frame #2 {
        # "Выключение происходит не быстро, поскольку есть особенность"
        n432 = local read "STAB+15"() -> (w850:bool)
        n433 = local read "STAB-15"() -> (w849:bool)
        n434 = local read "R_LOW"() -> (w847:bool)
        n435 = local read "VSUB"() -> (w848:bool)
        n436 = local read "ADC"() -> (w856:bool)
        n437 = local read "VDD"() -> (w853:bool)
        n438 = local read "ESD"() -> (w854:bool)
        n439 = local read "LED"() -> (w851:bool)
        n440 = local read "OG"() -> (w852:bool)
        n441 = local read "RD"() -> (w855:bool)
        n442 = Compound Arithmetic op=OR(w856, w855, w854, w853, w852, w851, w850, w849, w848, w847, "SIM_SEL") -> (w845:bool)
        n443 = case shown="True" w845 {
          tunnel: [w857 w859] -> w844
          tunnel: w843 -> [_ w858]
          frame False {
            n444 = local read "Стоп"() -> (w857:bool)
          }
          frame True {
            n445 = flat-sequence {
              tunnel: w858 -> [w860]
              tunnel: [w864] -> w859
              frame #0 {
                n446 = local write "Питание"(FALSE ("Питание")) -> ()
                n447 = xnode "Read/Write Control"("FPGA VI Reference In"=w860, "Линейки"=FALSE) -> ()  [unwired: 1 in, 2 out]
              }
              frame #1 {
                n448 = Wait (ms)(milliseconds to wait=u32 300) -> ()  [unwired: 1 out]
              }
              frame #2 {
                n449 = local write "Питание"(TRUE ("Питание")) -> ()
                n450 = local read "Стоп"() -> (w864:bool)
              }
            }
          }
        }
      }
    }
    n451 = Wait (ms)(milliseconds to wait=u32 1) -> ()  [unwired: 1 out]
  }
  n452 = while {
    shift-right: ["SAVE"] -> _
    shift-left: _ -> [w884]
    tunnel: w4 -> [_]
    stop <- w885 stop-if-true
    n453 = local read "Номер SUB"() -> (w879:u16)
    n454 = local read "17860?"() -> (w873:u16)
    n455 = local read "С_1265?"() -> (w881:u16)
    n456 = Greater?(x="SAVE", y=w884) -> (0:w883:bool)
    n457 = To Unsigned Long Integer(number=w873) -> (unsigned 32bit integer=w867:u32)
    n458 = Decrement(x=w879) -> (x-1=w878:u16)
    n459 = Decrement(x=w881) -> (x-1=w880:u16)
    n460 = Reciprocal(x="Частота, МГц?") -> (1/x=w868:dbl)
    n461 = Subtract(x=w880, y=w878) -> (x-y=w872:u16)
    n462 = Multiply(x=w868, y=w867) -> (x*y=w866:dbl)
    n463 = To Unsigned Long Integer(number=w872) -> (unsigned 32bit integer=w871:u32)
    n464 = local read "Между кадрами, мс"() -> (w876:u16)
    n465 = Multiply(x=w866, y=w871) -> (x*y=w870:dbl)
    n466 = local read "Стоп"() -> (w885:bool)
    n467 = Divide(x=w870, y=u32 1000) -> (x/y=w875:dbl)
    n468 = Add(x=w876, y=w875) -> (x+y=w874:dbl)
    "Тнак, мс" <- w874
    n469 = case shown="True" w883 {
      tunnel: w874 -> [_ w888]
      frame False {
        n470 = Wait (ms)(milliseconds to wait=u32 25) -> ()  [unwired: 1 out]
      }
      frame True {
        w889 = i16 0 ("width (-)")
        w901 = "_"
        n471 = local read "Номер образца"() -> (w892:string)
        n472 = local read "Температура"() -> (w895:string)
        n473 = Concatenate Strings("Темп. = " ("string"), w895) -> (w893:string)
        n474 = Get Date/Time In Seconds() -> (seconds since 1Jan1904=w917:timestamp)
        n475 = Number To Fractional String(number=w888, width (-)=w889, precision (6)=w889) -> (F-format string=w902:string)  [unwired: 1 in]
        n476 = Concatenate Strings("Образец_" ("string"), w892) -> (w890:string)
        n477 = Format Date/Time String(time format string (%c)="%H.%M.%S", seconds (now)=w917) -> (date/time string=w921:string)  [unwired: 1 in]
        n478 = Select(t="Светло", s="Светлый (T)\nТемный (F)", f="Темно") -> (s? t:f=w918:string)
        n479 = Build Path(base path="Frames", name or relative path=w890) -> (appended path=w912:path)
        n480 = call <vilib>:"Check if File or Folder Exists.vi"("path"=w912) -> ("file or folder exists?"=w911:bool, "dup path"=w910:path)  [unwired: 8 in, 1 out]
        n481 = local read "Image"() -> (w904:T2)
        n482 = Concatenate Strings(w921, w901, "ПРИМЕЧАНИЕ", w901, "Тн(мс)=" ("string"), w902, ".tiff" ("element")) -> (w920:string)
        n483 = case shown="False" w911 {
          tunnel: w910 -> [w930 w931]
          tunnel: [w929 w931] -> w897
          frame False {
            n484 = Create Folder(path (use dialog)=w930) -> (created path=w929:path)  [unwired: 2 in, 2 out]
          }
          frame True {
          }
        }
        n485 = Build Path(base path=w897, name or relative path=w893) -> (appended path=w898:path)
        n486 = call <vilib>:"Check if File or Folder Exists.vi"("path"=w898) -> ("file or folder exists?"=w899:bool, "dup path"=w900:path)  [unwired: 8 in, 1 out]
        n487 = case shown="False" w899 {
          tunnel: w900 -> [w924 w925]
          tunnel: [w923 w925] -> w896
          frame False {
            n488 = Create Folder(path (use dialog)=w924) -> (created path=w923:path)  [unwired: 2 in, 2 out]
          }
          frame True {
          }
        }
        n489 = Build Path(base path=w896, name or relative path=w918) -> (appended path=w913:path)
        n490 = call <vilib>:"Check if File or Folder Exists.vi"("path"=w913) -> ("file or folder exists?"=w914:bool, "dup path"=w915:path)  [unwired: 8 in, 1 out]
        n491 = case shown="False" w914 {
          tunnel: w915 -> [w927 w928]
          tunnel: [w926 w928] -> w919
          frame False {
            n492 = Create Folder(path (use dialog)=w927) -> (created path=w926:path)  [unwired: 2 in, 2 out]
          }
          frame True {
          }
        }
        n493 = Build Path(base path=w919, name or relative path=w920) -> (appended path=w916:path)
        n494 = call-poly "IMAQ Write File 2"("File Path"=w916, "Image"=w904) -> ()  [unwired: 8 in, 2 out]
      }
    }
  }
  n495 = while {
    tunnel: w4 -> [_]
    shift-right: [w941] -> _
    shift-left: _ -> [w942]
    stop <- w944 stop-if-true
    n496 = local read "Стоп"() -> (w944:bool)
    n497 = local read "Картинка"() -> (w941:bool)
    n498 = Wait (ms)(milliseconds to wait=u32 5) -> ()  [unwired: 1 out]
    n499 = Greater?(x=w941, y=w942) -> (0:w940:bool)
    n500 = Or(x=w940, y="Расчет") -> (x .or. y?=w938:bool)
    n501 = case shown="True" w938 {
      frame False {
      }
      frame True {
        # "ГОР"
        # "ВЕРТ"
        # "X1"
        # "Y1"
        n502 = local read "Analis"() -> (w1005:u16[][])
        n503 = To Double Precision Float(number=w1005) -> (double precision float=w953:dbl[][])
        n504 = property on="Image" class="ImageControl"() -> ("ROI"=w1043:T7)  [unwired: 2 in, 2 out]
        n505 = for {
          N: 1200 -> [_]
          tunnel: w953 -> [w1088]
          tunnel: [w1082] -> w1011 mode=indexing
          tunnel: 1635 -> [w1081]
          i -> [w1087]
          n506 = Add(x=20, y=w1087) -> (x+y=w1085:i32)
          n507 = Index Array(array=w1088, index (row)=w1085) -> (element=w1084:dbl[])  [unwired: 1 in]
          n508 = Delete From Array(array=w1084, length=w1081, index=37) -> (deleted portion=w1082:dbl[])  [unwired: 1 out]
        }
        n509 = To Double Precision Float(number=w1005) -> (double precision float=w1006:dbl[][])
        n510 = Unbundle By Name(w1043) -> ("Contours"=w1042:T8)
        n511 = Index Array(array=w1042, index=0) -> (element=w1040:T9)
        n512 = Unbundle By Name(w1040) -> ("Points"=w1039:i32[])
        n513 = Index Array(array=w1039, index=0) -> (element=w1033:i32)
        n514 = Index Array(array=w1039, index=1) -> (element=w1031:i32)
        n515 = Index Array(array=w1039, index=2) -> (element=w1034:i32)
        n516 = Index Array(array=w1039, index=3) -> (element=w1032:i32)
        n517 = local read "2/4 V"() -> (w1007:enum16{"2V", "4V"})
        n518 = Subtract(x=w1034, y=w1033) -> (x-y=w1029:i32)
        n519 = case shown="\"4V\"" w1007 {
          tunnel: [2000 4000] -> w1008
          frame "2V", Default {
          }
          frame "4V" {
          }
        }
        n520 = Subtract(x=w1032, y=w1031) -> (x-y=w1028:i32)
        n521 = for {
          N: w1029 -> [_]
          tunnel: w1033 -> [w1111]
          tunnel: w1031 -> [w1108]
          tunnel: w1028 -> [w1107]
          tunnel: w1006 -> [w1110]
          shift-right: [w1103] -> w1027
          shift-left: u64 0 -> [w1104]
          tunnel: [w1102] -> w1013 mode=indexing
          i -> [w1112]
          n522 = Add(x=w1111, y=w1112) -> (x+y=w1101:i32)
          n523 = Index Array(array=w1110, index (col)=w1101) -> (element=w1109:dbl[])  [unwired: 1 in]
          n524 = Delete From Array(array=w1109, length=w1107, index=w1108) -> (deleted portion=w1102:dbl[])  [unwired: 1 out]
          n525 = for {
            tunnel: w1102 -> [w1115] mode=indexing
            shift-right: [w1113] -> w1105
            shift-left: u64 0 -> [w1114]
            n526 = Add(x=w1115, y=w1114) -> (x+y=w1113:dbl)
          }
          n527 = Add(x=w1105, y=w1104) -> (x+y=w1103:dbl)
        }
        n528 = Multiply(x=w1029, y=w1028) -> (x*y=w983:i32)
        n529 = Index Array(array=w953, index (row)=13 ("disabled index (col)")) -> (element=w995:dbl[])  [unwired: 1 in]
        n530 = Divide(x=w1027, y=w983) -> (x/y=w982:dbl)
        n531 = local read "2/4 V"() -> (w1024:enum16{"2V", "4V"})
        n532 = for {
          tunnel: w1013 -> [w1092] mode=indexing
          tunnel: w982 -> [w1091]
          shift-right: [w1090] -> w1022
          shift-left: 0.0 -> [w1089]
          n533 = for {
            tunnel: w1092 -> [w1097] mode=indexing
            tunnel: w1091 -> [w1098]
            shift-right: [w1093] -> w1090
            shift-left: w1089 -> [w1094]
            n534 = Subtract(x=w1097, y=w1098) -> (x-y=w1096:dbl)
            n535 = Square(x=w1096) -> (x^2=w1095:dbl)
            n536 = Add(x=w1094, y=w1095) -> (x+y=w1093:dbl)
          }
        }
        n537 = Delete From Array(array=w995, length=1635, index=37) -> (deleted portion=w992:dbl[])  [unwired: 1 out]
        n538 = Divide(x=w982, y=65536.0) -> (x/y=w1025:dbl)
        n539 = Array Size(array=w992) -> (size(s)=w990:i32)
        n540 = case shown="\"4V\"" w1024 {
          tunnel: [2000 4000] -> w1012
          frame "2V", Default {
          }
          frame "4V" {
          }
        }
        n541 = Multiply(x=w1012, y=w1025) -> (x*y=w996:dbl)
        "Vout, мВ" <- w996
        n542 = Multiply(x=w996, y=5.0) -> (x*y=w997:dbl)
        n543 = Divide(x=w996, y=5.0) -> (x/y=w999:dbl)
        n544 = for {
          tunnel: w1011 -> [w1065] mode=indexing
          tunnel: w997 -> [w1064]
          tunnel: w999 -> [w1063]
          tunnel: w1008 -> [w1062]
          shift-right: [w1058] -> w1001
          shift-left: u32 0 -> [w1060]
          shift-right: [w1059] -> w1002
          shift-left: u32 0 -> [w1061]
          n545 = for {
            tunnel: w1065 -> [w1078] mode=indexing
            tunnel: w1064 -> [w1080]
            tunnel: w1063 -> [w1079]
            tunnel: w1062 -> [w1075]
            shift-right: [w1067] -> w1059
            shift-left: w1061 -> [w1069]
            shift-right: [w1066] -> w1058
            shift-left: w1060 -> [w1068]
            n546 = Divide(x=w1078, y=65536.0) -> (x/y=w1076:dbl)
            n547 = Multiply(x=w1075, y=w1076) -> (x*y=w1074:dbl)
            n548 = Greater?(x=w1074, y=w1080) -> (0:w1070:bool)
            n549 = Less?(x=w1074, y=w1079) -> (x < y?=w1073:bool)
            n550 = Increment(x=w1069) -> (x+1=w1072:u32)
            n551 = Increment(x=w1068) -> (x+1=w1071:u32)
            n552 = Select(t=w1072, s=w1070, f=w1069) -> (s? t:f=w1067:u32)
            n553 = Select(t=w1071, s=w1073, f=w1068) -> (s? t:f=w1066:u32)
          }
        }
        "Nбд" <- w1002
        "Nчд" <- w1001
        n554 = for {
          tunnel: w992 -> [w1055] mode=indexing
          shift-right: [w1053] -> w991
          shift-left: 0.0 -> [w1054]
          n555 = Add(x=w1055, y=w1054) -> (x+y=w1053:dbl)
        }
        n556 = Divide(x=w991, y=w990) -> (x/y=w977:dbl)
        n557 = Index Array(array=w953, index (row)=1252 ("disabled index (col)")) -> (element=w984:dbl[])  [unwired: 1 in]
        n558 = Delete From Array(array=w984, length=1635, index=37) -> (deleted portion=w987:dbl[])  [unwired: 1 out]
        n559 = Divide(x=w1022, y=w982) -> (x/y=w1021:dbl)
        n560 = Index Array(array=w953, index (col)=1676 ("disabled index (col)")) -> (element=w955:dbl[])  [unwired: 1 in]
        n561 = Index Array(array=w953, index (col)=37 ("disabled index (col)")) -> (element=w968:dbl[])  [unwired: 1 in]
        n562 = Square Root(x=w1021) -> (sqrt(x)=w1019:dbl)
        n563 = for {
          tunnel: w987 -> [w1052] mode=indexing
          shift-right: [w1050] -> w988
          shift-left: 0.0 -> [w1051]
          n564 = Add(x=w1052, y=w1051) -> (x+y=w1050:dbl)
        }
        n565 = Delete From Array(array=w955, length=1200, index=20) -> (deleted portion=w958:dbl[])  [unwired: 1 out]
        n566 = Delete From Array(array=w968, length=1200, index=20) -> (deleted portion=w965:dbl[])  [unwired: 1 out]
        n567 = Divide(x=w1019, y=65536.0) -> (x/y=w1018:dbl)
        n568 = Array Size(array=w987) -> (size(s)=w989:i32)
        n569 = Multiply(x=w1018, y=w1012) -> (x*y=w1017:dbl)
        "DSNU, мВ, p-p" <- w1017
        n570 = for {
          tunnel: w958 -> [w1046] mode=indexing
          shift-right: [w1044] -> w959
          shift-left: 0.0 -> [w1045]
          n571 = Add(x=w1046, y=w1045) -> (x+y=w1044:dbl)
        }
        n572 = for {
          tunnel: w965 -> [w1049] mode=indexing
          shift-right: [w1047] -> w964
          shift-left: 0.0 -> [w1048]
          n573 = Add(x=w1049, y=w1048) -> (x+y=w1047:dbl)
        }
        n574 = Divide(x=w988, y=w989) -> (x/y=w973:dbl)
        n575 = Divide(x=w1017, y=w996) -> (x/y=w1016:dbl)
        n576 = Multiply(x=w1016, y=100.0) -> (x*y=→"PRNU, %":dbl)
        n577 = Array Size(array=w958) -> (size(s)=w960:i32)
        n578 = Array Size(array=w965) -> (size(s)=w963:i32)
        n579 = Subtract(x=w973, y=w977) -> (x-y=w976:dbl)
        n580 = Divide(x=w976, y=1239.0) -> (x/y=w974:dbl)
        n581 = Divide(x=w974, y=w973) -> (x/y=w971:dbl)
        n582 = Subtract(x=1.0, y=w971) -> (x-y=→"Ev":dbl)
        n583 = Divide(x=w959, y=w960) -> (x/y=w952:dbl)
        n584 = Divide(x=w964, y=w963) -> (x/y=w945:dbl)
        n585 = Subtract(x=w945, y=w952) -> (x-y=w951:dbl)
        n586 = Divide(x=w951, y=1639.0) -> (x/y=w946:dbl)
        n587 = Divide(x=w946, y=w945) -> (x/y=w947:dbl)
        n588 = Subtract(x=1.0, y=w947) -> (x-y=→"Eh":dbl)
      }
    }
    n589 = local read "DSNU, мВ, p-p"() -> (w932:dbl)
    n590 = Divide(x="Uнас, мВ", y=w932) -> (x/y=w935:dbl)
    n591 = Logarithm Base 10(1:w935) -> (0:w936:dbl)
    n592 = Multiply(x=w936, y=20.0) -> (x*y=→"D, дБ":dbl)
  }
  n593 = call <instrlib>:"niDCPower Close.vi"("instrument handle"=w16) -> ()  [unwired: 10 in, 1 out]
  n594 = call <instrlib>:"niDCPower Close.vi"("instrument handle"=w14) -> ()  [unwired: 10 in, 1 out]
  n595 = call <instrlib>:"niDCPower Close.vi"("instrument handle"=w13) -> ()  [unwired: 10 in, 1 out]
  n596 = call <instrlib>:"niDCPower Close.vi"("instrument handle"=w15) -> ()  [unwired: 10 in, 1 out]
  n597 = xnode "Close FPGA VI Reference"("FPGA VI Reference In"=w5) -> ()  [unwired: 1 in, 1 out]
